vi "TS Manager_wo TS.vi"(11 "notifier":refnum<notifier>) -> ()   [LabVIEW 2025, in "Config Tool.lvlib"]
doc: "This is the main VI for the configuration editor.Copyright 2017 National Instruments Corporation\n\nLicensed under the Apache License, Version 2.0 (the \"License\"); you may not use this file except in compliance with the License. You may obtain a copy of the License at http://www.apache.org/licenses/LICENSE-2.0\nUnless required by applicable law or agreed to in writing, software distributed under the License is distributed on an \"AS IS\" BASIS, WITHOUT WARRANTIES OR CONDITIONS OF ANY KIND, either express or implied. See the License for the specific language governing permissions and limitations under the License."
uses:
  Controls/StateCluster.ctl
  Users/Public/Documents/Sandia National Labs/TSS Plugin/CEF.lvlibp/Repository/CEF_Repository.lvclass
  Users/Public/Documents/Sandia National Labs/TSS Plugin/CEF.lvlibp/Node/NodeRef.ctl
  Users/Public/Documents/Sandia National Labs/TSS Plugin/CEF.lvlibp/Node/CEF_Node.lvclass
  Users/Public/Documents/Sandia National Labs/TSS Plugin/CEF.lvlibp/Node/StandardEvents.ctl
  Controls/FilePaths.ctl
  Users/Public/Documents/Sandia National Labs/TSS Plugin/CEF.lvlibp/glyph manager/glyph manager.ctl
  <vilib>/Utility/config.llb/Config Data RefNum.ctl
  Controls/AddMessage.ctl
  Controls/MoveMessage.ctl
  Users/Public/Documents/Sandia National Labs/TSS Plugin/CEF.lvlibp/hierarchy repo/CEF_HierarchyRepo.lvclass
  Users/Public/Documents/Sandia National Labs/TSS Plugin/System.lvlibp/System/System.lvclass
  Users/Public/Documents/Sandia National Labs/TSS Plugin/CEF.lvlibp/serializable node/CEF_serializable node.lvclass
  ce7dbd15-68e1-444f-b0a0-607e461cde1a.vi
  TestStandUI/Control Globals.vi
  Users/Public/Documents/Sandia National Labs/TSS Plugin/CEF.lvlibp/Node/ReadChildren.vi
  Users/Public/Documents/Sandia National Labs/TSS Plugin/CEF.lvlibp/Node/ReadNodeClass.vi
  Config Tool.lvlib
  C:/Users/Public/Documents/Sandia National Labs/TSS Plugin/CEF.lvlibp/Repository/CEF_Repository.lvclass
  C:/Users/Public/Documents/Sandia National Labs/TSS Plugin/CEF.lvlibp/hierarchy repo/CEF_HierarchyRepo.lvclass
  C:/Users/Public/Documents/Sandia National Labs/TSS Plugin/CEF.lvlibp/Node/CEF_Node.lvclass
  C:/Users/Public/Documents/Sandia National Labs/TSS Plugin/CEF.lvlibp/serializable node/CEF_serializable node.lvclass
  Users/Public/Documents/Sandia National Labs/TSS Plugin/CEF.lvlibp
  <vilib>/Utility/config.llb/NI_LVConfig.lvlib
panel:
  in  "Record":bool
  out "Time":dbl format="%<%H:%M:%S>t"
  in  "Initialize Engines":bool
  in  "File Menu":bool
  in  "TreeView":string(tree)="NID741343233"
  in  "TS Pane":bool
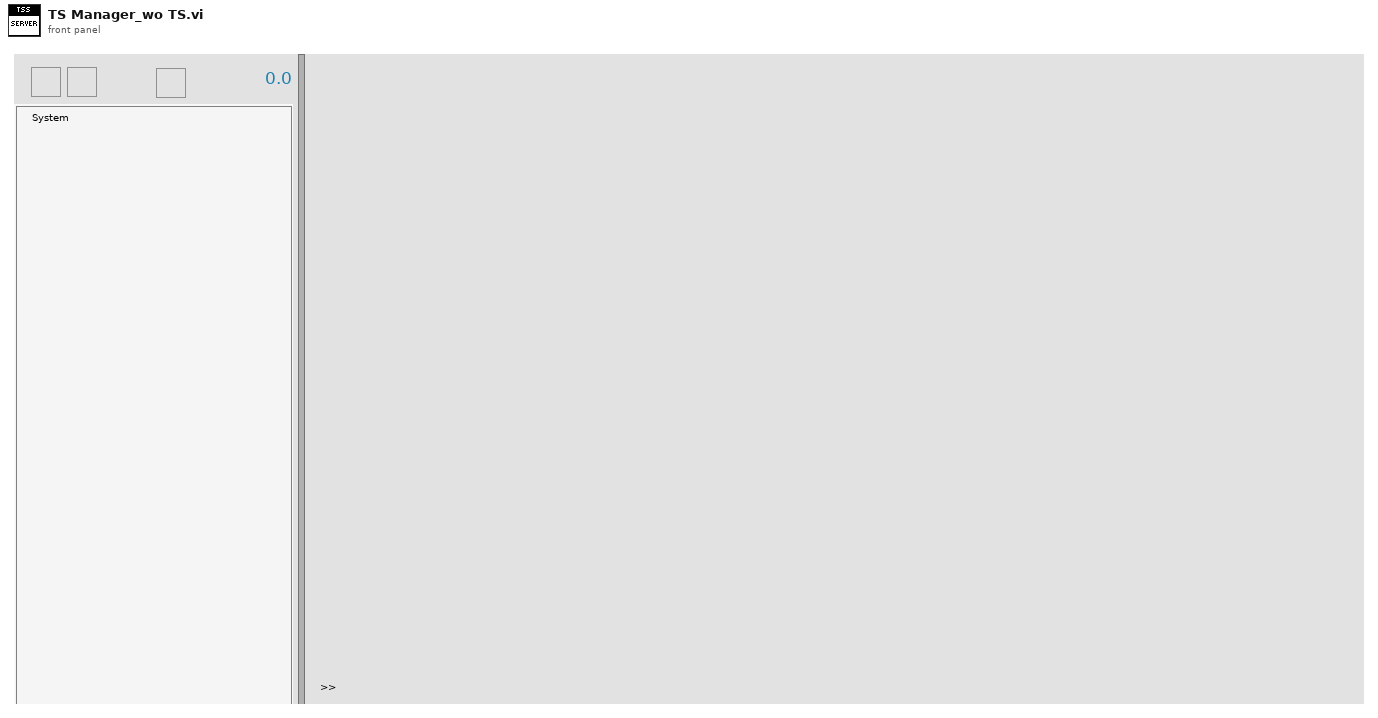
[diagram p1: front panel]
types:
  T1 = typedef "Config Tool.lvlib/StateCluster.ctl" = cluster{"repository":refnum<class "CEF_Repository.lvclass">, "root":T2, "standard events":T3, "paths":T4, "glyph manager":T5, "current path":path, "unsaved changes":bool, "menu":refnum<k9>, "Error Log":refnum<file>, "INI file ref":T6, "Record":bool, "tdms file":refnum<k34>}
  T2 = typedef "CEF.lvlibp/CEF_Node.lvclass/NodeRef.ctl" = refnum<data-value>
  T3 = typedef "CEF.lvlibp/CEF_Node.lvclass/StandardEvents.ctl" = cluster{"user event":refnum<user-event>, "node change":refnum<user-event>, "cache state":refnum<user-event>, "refresh UI":refnum<user-event>, "stop event":refnum<user-event>, "Quit App":refnum<user-event>}
  T4 = typedef "Config Tool.lvlib/FilePaths.ctl" = cluster{"Configuration":path, "Plugin":path, "Glyphs":path, "Data":path, "Error Log":path}
  T5 = typedef "CEF.lvlibp/glyph manager.ctl" = cluster{"search paths":path[], "glyph map":variant, "base glyphs":cluster{"image type":i32, "image depth":i32, "image":u8[], "mask":u8[], "colors":u32[], "Rectangle":cluster{"left":i16, "top":i16, "right":i16, "bottom":i16}}[], "desired overlays":string[]}
  T6 = typedef "NI_LVConfig.lvlib/Config Data RefNum.ctl" = refnum<k1>
  T7 = cluster{"user event":refnum<user-event>, "node change":refnum<user-event>, "cache state":refnum<user-event>, "refresh UI":refnum<user-event>, "stop event":refnum<user-event>, "Quit App":refnum<user-event>}
  T8 = typedef "Config Tool.lvlib/AddMessage.ctl" = cluster{"subNode":string, "Node ID":string}
  T9 = typedef "Config Tool.lvlib/MoveMessage.ctl" = cluster{"node ref":T2, "new parent":T2, "Index":i32}
  T10 = cluster{"Message Name":string, "data string":string}
  T11 = typedef "LVPoint32TypeDef.ctl" = cluster{"Horizontal":i32, "Vertical":i32}
  T12 = cluster{"data name":string, "drag data":variant}[]
  T13 = cluster{"removable":bool, "movable":bool, "duplicate":bool}
  T14 = cluster{"message name":string, "data string":string}
  T15 = enum16{"Start Timer", "Read Time", "Pause", "Resume"}
  T16 = enum16{"open", "open or create", "create or replace", "create", "open (read-only)"}
  T17 = cluster{"search paths":path[], "glyph map":variant, "base glyphs":cluster{"image type":i32, "image depth":i32, "image":u8[], "mask":u8[], "colors":u32[], "Rectangle":cluster{"left":i16, "top":i16, "right":i16, "bottom":i16}}[], "desired overlays":string[]}
  T18 = cluster{"ID":string, "parent ID":string, "node type":string, "text":string, "additional text":string, "glyph":string, "depth":i32, "glyph overlay":string}[]
  T19 = cluster{"ID":string, "parent ID":string, "node type":string, "text":string, "additional text":string, "glyph":string, "depth":i32, "glyph overlay":string}
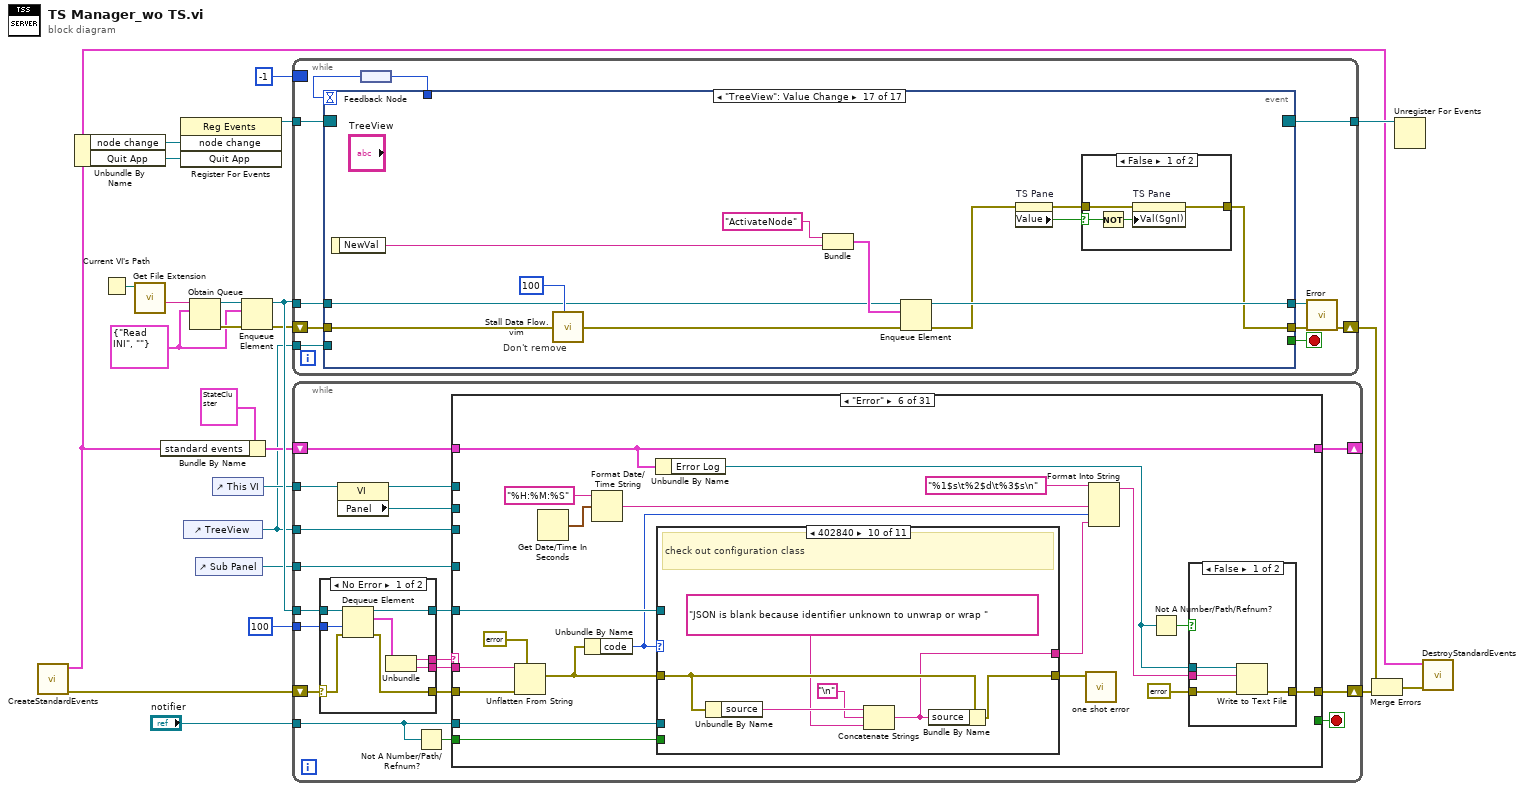
[diagram p0: block diagram]
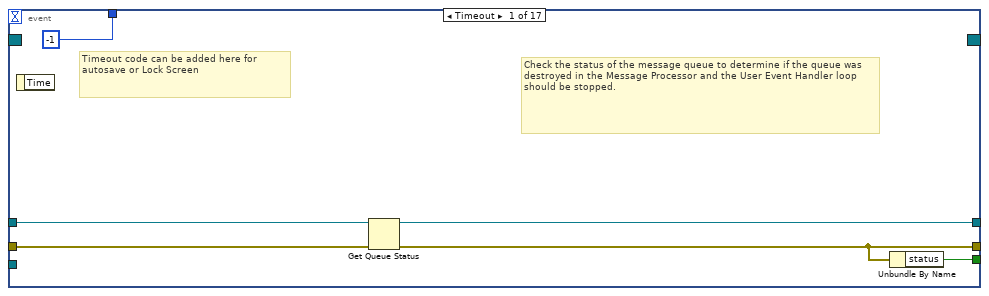
[diagram p2: hidden frame]
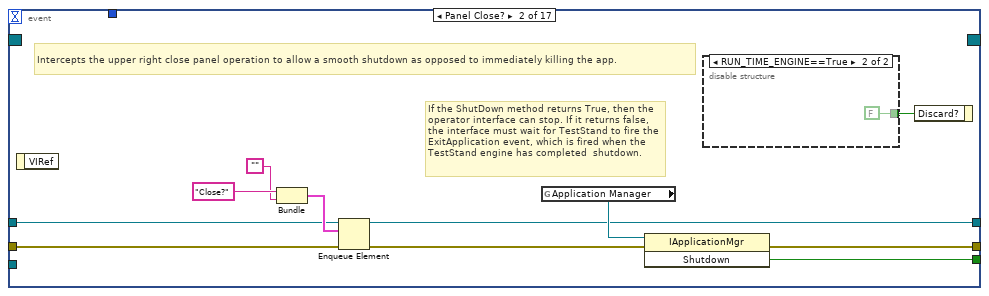
[diagram p3: hidden frame]
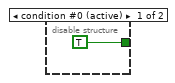
[diagram p4: hidden frame]
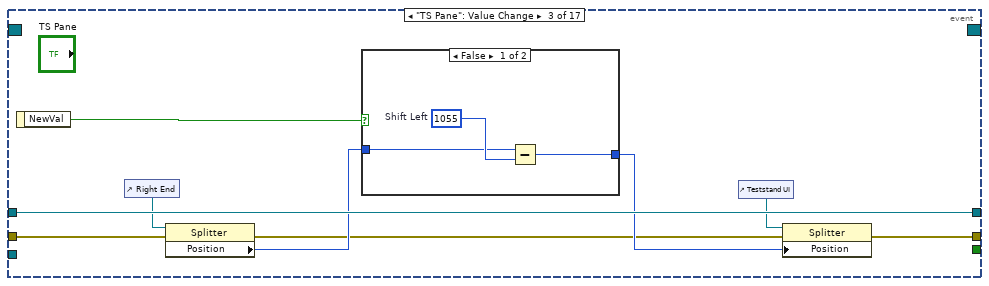
[diagram p5: hidden frame]
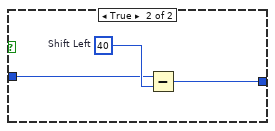
[diagram p6: hidden frame]
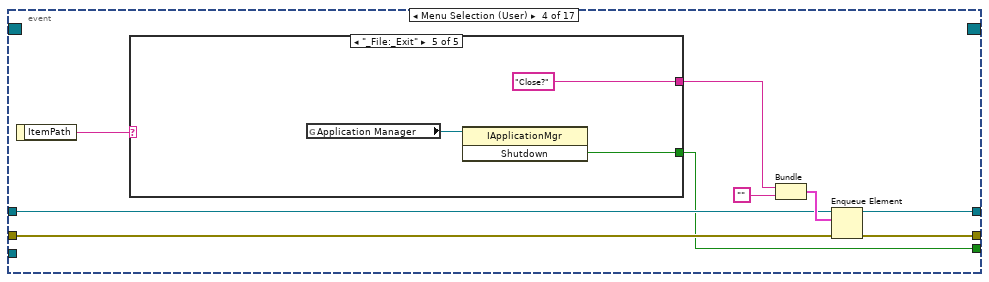
[diagram p7: hidden frame]
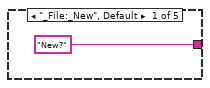
[diagram p8: hidden frame]
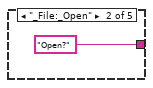
[diagram p9: hidden frame]
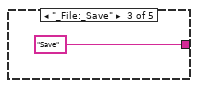
[diagram p10: hidden frame]
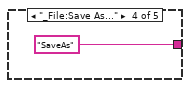
[diagram p11: hidden frame]
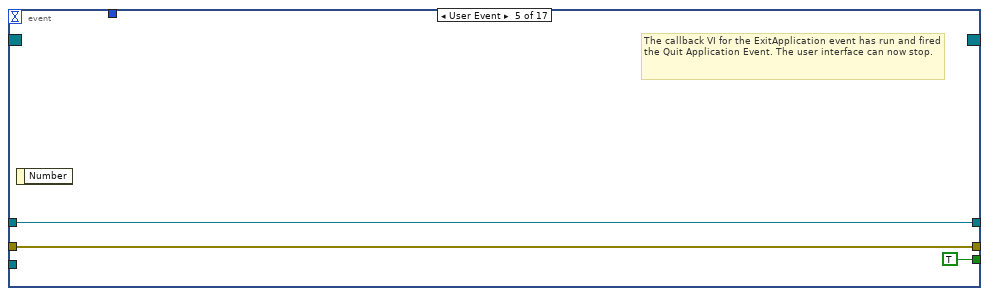
[diagram p12: hidden frame]
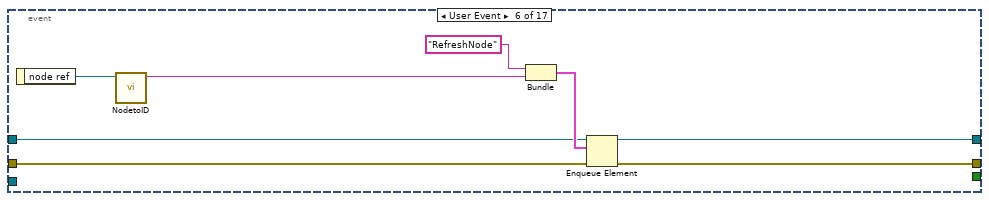
[diagram p13: hidden frame]
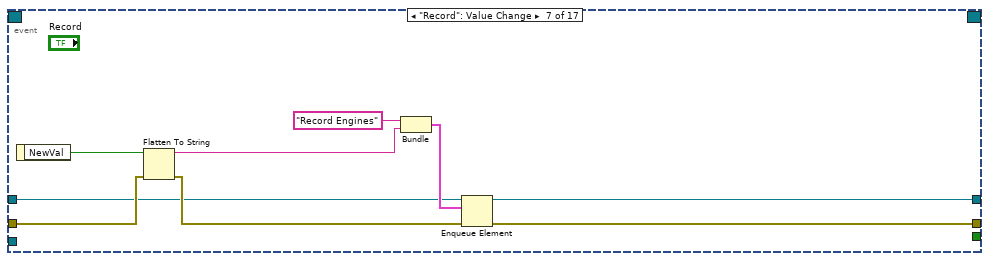
[diagram p14: hidden frame]
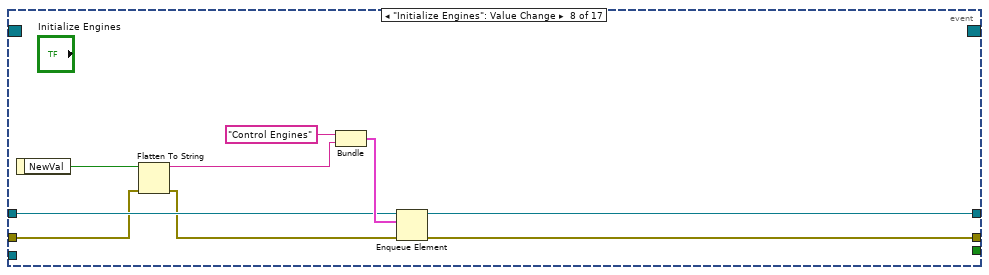
[diagram p15: hidden frame]
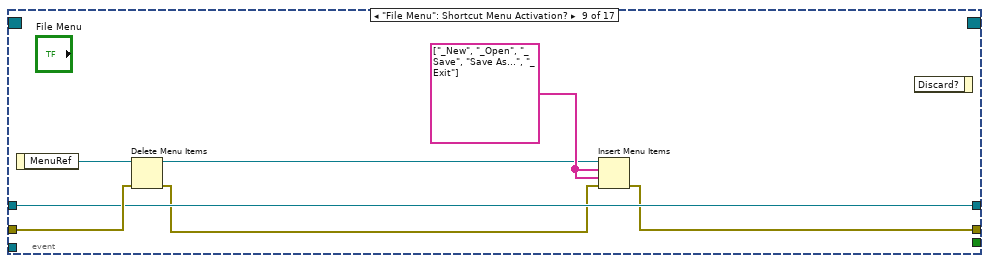
[diagram p16: hidden frame]
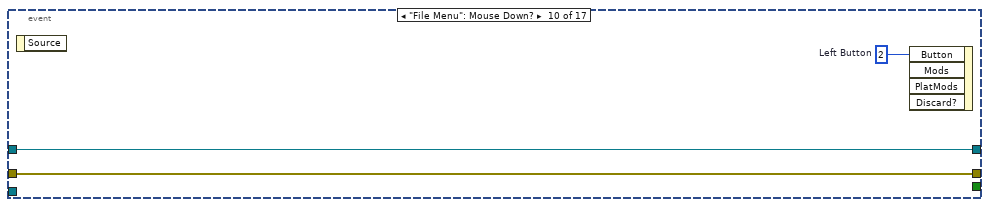
[diagram p17: hidden frame]
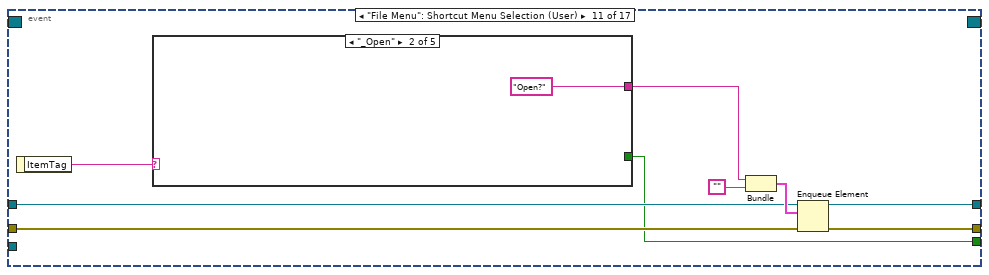
[diagram p18: hidden frame]
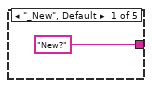
[diagram p19: hidden frame]
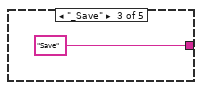
[diagram p20: hidden frame]
diagram:
  w10 = cluster{"message":string, "string":string} {"message"="Read INI", "string"=""}
  n1 = call "CreateStandardEvents.vi"() -> ("error out"=w14:errorcluster, "standard events"=w16:T7)  [unwired: 10 in]
  n2 = Unbundle By Name(w16) -> ("node change"=w15:refnum<user-event>, "Quit App"=w1:refnum<user-event>)
  n3 = Current VI's Path() -> (path=w21:path)
  n4 = call <vilib>:"Get File Extension.vi"("file"=w21) -> ("filename without extension"=w11:string)  [unwired: 6 in, 4 out]
  n5 = Bundle By Name(cluster=T1 {"repository"=refnum, "root"=refnum, "standard events"={"user event"=refnum, "node change"=refnum, "cache state"=refnum, "refresh UI"=refnum, "stop event"=refnum, "Quit App"=refnum}, "paths"={"Configuration"=path "", "Plugin"=path "", "Glyphs"=path "", "Data"=path "", "Error Log"=path ""}, "glyph manager"={"search paths"=[], "glyph map"=variant, "base glyphs"=[], "desired overlays"=[]}, "current path"=path "", "unsaved changes"=FALSE, "menu"=refnum, "Error Log"=refnum, "INI file ref"=refnum, "Record"=FALSE, "tdms file"=refnum} ("state cluster"), "standard events"=w16) -> (w4:T1)
  n6 = register-events(w15, w1) -> (reference out=w2:refnum<event-registration>)  [unwired: 2 in, 1 out]
  n7 = control-ref of="TreeView"() -> (w3:refnum<vi>)
  n8 = Obtain Queue(name (unnamed)=w11, element data type=w10) -> (queue out=w12:refnum<queue>, error out=w13:errorcluster)  [unwired: 3 in, 1 out]
  n9 = control-ref of="Sub Panel"() -> (w5:refnum<vi>)
  n10 = control-ref of="This VI"() -> (w6:refnum<vi>)
  n11 = Enqueue Element(queue=w12, element=w10, error in (no error)=w13) -> (queue out=w9:refnum<queue>, error out=w8:errorcluster)  [unwired: 1 in, 1 out]
  n12 = while "User Interface Event Handler" {
    tunnel: w9 -> [w34]
    tunnel: w3 -> [w29]
    tunnel: w2 -> [w28]
    tunnel: [w27] -> w17
    border: -1 -> [_]
    shift-right: [w31] -> w22
    shift-left: w8 -> [w35]
    stop <- w33 stop-if-true
    n13 = feedback #1() -> (w25:i32)
    n14 = event shown="[16] \"TreeView\": Value Change" {
      selector: w28 -> [_ _ _ _ _ _ _ _ _ _ _ _ _ _ _ _ _]
      dyn-events: [_ _ _ _ _ _ _ _ _ _ _ _ _ _ _ _ _] -> w27
      timeout: w25 -> [_ _ _ _ _ _ _ _ _ _ _ _ _ _ _ _ _]
      tunnel: [w36 w49 _ w71 TRUE ("Shutdown") _ _ _ _ _ w127 _ _ _ _ _ _] -> w33
      tunnel: [w37 w51 w62 w78 w90 w97 w101 w108 w117 w124 w128 w159 w182 w211 w239 w250 w279] -> w32
      tunnel: w35 -> [w38 w45 w57 w72 w90 w91 w103 w110 w123 w124 w129 w150 w181 w210 w237 w251 w290]
      tunnel: w34 -> [w41 w44 w64 w73 w89 w93 w102 w114 w121 w125 w131 w148 w177 w209 w236 w245 w284]
      tunnel: [w40 w43 w64 w77 w89 w92 w100 w113 w121 w125 w130 w148 w176 w209 w236 _ w283] -> w30
      tunnel: w29 -> [_ _ _ _ _ _ _ _ _ _ _ w146 _ _ _ _ _]
      tunnel: [-1 _ _ _ _ _ _ _ _ _ _ _ _ _ _ _ _] -> w26
      event Timeout {
        # "Check the status of the message queue to determine if the queue was destroyed in the Message Processor and the User Event Handler loop should be stopped."
        # "Timeout code can be added here for autosave or Lock Screen"
        n15 = event-data() -> ()  [unwired: 1 in, 1 out]
        n16 = Get Queue Status(queue=w41, error in (no error)=w38) -> (queue out=w40:refnum<queue>, error out=w37:errorcluster)  [unwired: 1 in, 6 out]
        n17 = Unbundle By Name(w37) -> ("status"=w36:bool)
      }
      event Panel Close? {
        # "If the ShutDown method returns True, then the operator interface can stop. If it returns false, the interface must wait for TestStand to fire the ExitApplication event, which is fired when the TestStand engine has completed  shutdown."
        # "Intercepts the upper right close panel operation to allow a smooth shutdown as opposed to immediately killing the app."
        n18 = event-data() -> ()  [unwired: 1 in, 1 out]
        n19 = Bundle("Close?", "") -> (w48:cluster{string, string})  [unwired: 1 in]
        n20 = Enqueue Element(queue=w44, element=w48, error in (no error)=w45) -> (queue out=w43:refnum<queue>, error out=w42:errorcluster)  [unwired: 1 in, 1 out]
        n21 = global read "Control Globals.vi" "Application Manager"() -> (w50:refnum<k7>)
        n22 = global read "Control Globals.vi" "Application Manager"() -> (w52:refnum<k7>)
        n23 = invoke class="IApplicationMgr" method="Shutdown"(reference=w50, error in=w42) -> ()  [unwired: 1 in, 3 out]
        n24 = invoke class="IApplicationMgr" method="Shutdown"(reference=w52) -> (error out=w51:errorcluster, "Shutdown"=w49:bool)  [unwired: 2 in, 1 out]
        n25 = disable-structure shown="RUN_TIME_ENGINE==True" {
          disable-tunnel: [TRUE FALSE] -> w53
          frame condition #0 (active) {
          }
          frame condition #1 {
          }
        }
        n26 = event-data("Discard?"=w53) -> ()  [unwired: 1 in, 1 out]
      }
      event "TS Pane": Value Change {
        n27 = event-data() -> ("NewVal"=w60:bool)  [unwired: 1 in]
        n28 = control-ref of="Right End"() -> (w61:refnum<vi>)
        n29 = property class="Splitter"(reference=w61, error in=w57) -> (error out=w56:errorcluster, "Position"=w59:i32)  [unwired: 1 out]
        n30 = case shown="False" w60 {
          tunnel: w59 -> [w66 w69]
          tunnel: [w65 w68] -> w58
          frame False {
            w67 = 1055  # Shift Left
            n31 = Subtract(x=w66, y=w67) -> (x-y=w65:i32)
          }
          frame True {
            w70 = 40  # Shift Left
            n32 = Subtract(x=w69, y=w70) -> (x-y=w68:i32)
          }
        }
        n33 = control-ref of="Teststand UI"() -> (w63:refnum<vi>)
        n34 = property class="Splitter"(reference=w63, error in=w56, "Position"=w58) -> (error out=w62:errorcluster)  [unwired: 1 out]
      }
      event Menu Selection (User) {
        n35 = event-data() -> ("ItemPath"=w79:string)  [unwired: 1 in]
        n36 = case shown="\"_File:_Exit\"" w79 {
          tunnel: ["New?" ("Message Name") "Open?" ("Message Name") "Save" ("Message Name") "SaveAs" ("Message Name") "Close?" ("Message Name")] -> w75
          tunnel: [_ _ _ _ w84] -> w71
          frame "_File:_New", Default {
          }
          frame "_File:_Open" {
          }
          frame "_File:_Save" {
          }
          frame "_File:Save As..." {
          }
          frame "_File:_Exit" {
            n37 = global read "Control Globals.vi" "Application Manager"() -> (w85:refnum<k7>)
            n38 = global read "Control Globals.vi" "Application Manager"() -> (w86:refnum<k7>)
            n39 = invoke class="IApplicationMgr" method="Shutdown"(reference=w85) -> ("Shutdown"=w84:bool)  [unwired: 2 in, 2 out]
            n40 = invoke class="IApplicationMgr" method="Shutdown"(reference=w86) -> ()  [unwired: 2 in, 3 out]
          }
        }
        n41 = Bundle("Message Name"=w75, "") -> (w74:cluster{"Message Name":string, string})  [unwired: 1 in]
        n42 = Enqueue Element(queue=w73, element=w74, error in (no error)=w72) -> (queue out=w77:refnum<queue>, error out=w78:errorcluster)  [unwired: 1 in, 1 out]
      }
      event User Event {
        # "The callback VI for the ExitApplication event has run and fired the Quit Application Event. The user interface can now stop."
        n43 = event-data() -> ()  [unwired: 1 in, 1 out]
      }
      event User Event {
        n44 = event-data() -> ("node ref"=w98:refnum<data-value>)  [unwired: 1 in]
        n45 = call "NodetoID.vi"("node ref"=w98) -> ("ID"=w94:string)  [unwired: 9 in, 1 out]
        n46 = Bundle("message name"="RefreshNode", "ID"=w94) -> (w95:cluster{"message name":string, "ID":string})  [unwired: 1 in]
        n47 = Enqueue Element(queue=w93, element=w95, error in (no error)=w91) -> (queue out=w92:refnum<queue>, error out=w97:errorcluster)  [unwired: 1 in, 1 out]
      }
      event "Record": Value Change {
        n48 = event-data() -> ("NewVal"=w99:bool)  [unwired: 1 in]
        n49 = Flatten To String(anything=w99, error in (no error)=w103) -> (data string=w105:string, error out=w104:errorcluster)  [unwired: 2 in, 1 out]
        n50 = Bundle("Message Name"="Record Engines", "data string"=w105) -> (w107:T10)  [unwired: 1 in]
        n51 = Enqueue Element(queue=w102, element=w107, error in (no error)=w104) -> (queue out=w100:refnum<queue>, error out=w101:errorcluster)  [unwired: 1 in, 1 out]
      }
      event "Initialize Engines": Value Change {
        n52 = event-data() -> ("NewVal"=w112:bool)  [unwired: 1 in]
        n53 = Flatten To String(anything=w112, error in (no error)=w110) -> (data string=w111:string, error out=w109:errorcluster)  [unwired: 2 in, 1 out]
        n54 = Bundle("Message Name"="Control Engines", "data string"=w111) -> (w116:T10)  [unwired: 1 in]
        n55 = Enqueue Element(queue=w114, element=w116, error in (no error)=w109) -> (queue out=w113:refnum<queue>, error out=w108:errorcluster)  [unwired: 1 in, 1 out]
      }
      event "File Menu": Shortcut Menu Activation? {
        w120 = string[] ["_New", "_Open", "_Save", "Save As...", "_Exit"] ("item names")
        n56 = event-data() -> ("MenuRef"=w122:refnum<k9>)  [unwired: 1 in]
        n57 = Delete Menu Items(6:w123, 9:w122) -> (0:w118:errorcluster, 3:w119:refnum<k9>)  [unwired: 2 in]
        n58 = Insert Menu Items(6:w118, 7:w120, 8:w120, 9:w119) -> (0:w117:errorcluster)  [unwired: 2 in, 2 out]
        n59 = event-data() -> ()  [unwired: 2 in, 1 out]
      }
      event "File Menu": Mouse Down? {
        w126 = u16 2  # Left Button
        n60 = event-data() -> ()  [unwired: 1 in, 1 out]
        n61 = event-data("Button"=w126) -> ()  [unwired: 4 in, 1 out]
      }
      event "File Menu": Shortcut Menu Selection (User) {
        n62 = event-data() -> ("ItemTag"=w135:string)  [unwired: 1 in]
        n63 = case shown="\"_Open\"" w135 {
          tunnel: ["New?" ("Message Name") "Open?" ("Message Name") "Save" ("Message Name") "SaveAs" ("Message Name") "Close?" ("Message Name")] -> w133
          tunnel: [_ _ _ _ w141] -> w127
          frame "_New", Default {
          }
          frame "_Open" {
          }
          frame "_Save" {
          }
          frame "Save As..." {
          }
          frame "_Exit" {
            n64 = global read "Control Globals.vi" "Application Manager"() -> (w142:refnum<k7>)
            n65 = global read "Control Globals.vi" "Application Manager"() -> (w143:refnum<k7>)
            n66 = invoke class="IApplicationMgr" method="Shutdown"(reference=w142) -> ("Shutdown"=w141:bool)  [unwired: 2 in, 2 out]
            n67 = invoke class="IApplicationMgr" method="Shutdown"(reference=w143) -> ()  [unwired: 2 in, 3 out]
          }
        }
        n68 = Bundle("Message Name"=w133, "") -> (w132:cluster{"Message Name":string, string})  [unwired: 1 in]
        n69 = Enqueue Element(queue=w131, element=w132, error in (no error)=w129) -> (queue out=w130:refnum<queue>, error out=w128:errorcluster)  [unwired: 1 in, 1 out]
      }
      event "TreeView": Shortcut Menu Activation? {
        n70 = event-data() -> ("MenuRef"=w149:refnum<k9>, "CtlRef"=w162:refnum<vi>, "Coords"=w161:T11)  [unwired: 1 in]
        n71 = invoke class="Tree (strict)" method="Point To Row Column"(reference=w162, "Point"=w161) -> ("Tag"=w160:string)  [unwired: 6 in, 7 out]
        n72 = property class="Tree (strict)"(reference=w146, error in=w150) -> (error out=w147:errorcluster, "Allow Editing Cells"=w145:bool)  [unwired: 1 out]
        n73 = call "IDtoNode.vi"("error in"=w147, "ID"=w160) -> ("error out"=w155:errorcluster, "invalid Id"=w153:bool, "node ref"=w158:refnum<data-value>)  [unwired: 7 in]
        n74 = Not(x=w153) -> (.not. x?=w144:bool)
        n75 = And(x=w144, y=w145) -> (x .and. y?=w152:bool)
        n76 = case shown="True" w152 {
          tunnel: w158 -> [_ w170]
          tunnel: w149 -> [_ w169]
          tunnel: [_ w168] -> w157
          tunnel: [_ w167] -> w156
          tunnel: w155 -> [w164 w166]
          tunnel: [w164 w166] -> w154
          tunnel: [TRUE ("Discard?") FALSE ("Discard?")] -> w151
          frame False {
          }
          frame True {
            n77 = in-place {
              in-place-border: w169 -> [w173]
              in-place-border: [w171] -> w168
              n78 = in-place-dvr #2(w170) -> (w175:refnum<class "CEF_Node.lvclass">, w172:errorcluster)
              n79 = call-dynamic "ShortcutMenu.vi"("error in"=w172, "menu ref in"=w173, "CEF_Node in"=w175) -> ("error out"=w171:errorcluster, "CEF_Node out"=w174:refnum<class "CEF_Node.lvclass">)  [unwired: 6 in, 1 out]
              n80 = in-place-dvr #2(w174) -> (w167:errorcluster)  [unwired: 1 out]
            }
          }
        }
        n81 = Merge Errors(w156, w157, w154) -> (w159:errorcluster)
        n82 = event-data("Discard?"=w151) -> ()  [unwired: 1 in, 1 out]
      }
      event "TreeView": Shortcut Menu Selection (User) {
        n83 = event-data() -> ("ItemPath"=w184:string, "CtlRef"=w187:refnum<vi>, "Coords"=w188:T11)  [unwired: 1 in]
        n84 = invoke class="Tree (strict)" method="Point To Row Column"(reference=w187, "Point"=w188) -> ("Tag"=w183:string)  [unwired: 6 in, 7 out]
        n85 = Match Pattern(string=w184, regular expression=":") -> (before substring=w186:string, after substring=w185:string)  [unwired: 1 in, 2 out]
        n86 = case shown="\"Export\"" w186 {
          selector: w186 -> [w192 _ _ _ _ _]
          tunnel: w185 -> [_ _ _ w202 _ _]
          tunnel: w183 -> [w193 w195 w197 w203 w205 w208]
          tunnel: ["CustomMenuAction" ("Message Name") "RemoveNode" ("Message Name") "Duplicate" ("Message Name") "AddNode" ("Message Name") "Import Engine" ("Message Name") "Export Engine" ("Message Name")] -> w179
          tunnel: [w190 w195 w197 w199 w205 w208] -> w180
          frame Default {
            # "Right click menu"
            n87 = Concatenate Strings(w192, ":" ("string"), w193) -> (w190:string)
          }
          frame "Remove" {
          }
          frame "Duplicate" {
          }
          frame "Add" {
            n88 = Bundle By Name(cluster=T8 {"subNode"="", "Node ID"=""} ("input cluster"), "subNode"=w202, "Node ID"=w203) -> (w200:T8)
            n89 = Flatten To String(anything=w200) -> (data string=w199:string)  [unwired: 3 in, 2 out]
          }
          frame "Import" {
          }
          frame "Export" {
          }
        }
        n90 = Bundle("Message Name"=w179, "Tag"=w180) -> (w178:cluster{"Message Name":string, "Tag":string})  [unwired: 1 in]
        n91 = Enqueue Element(queue=w177, element=w178, error in (no error)=w181) -> (queue out=w176:refnum<queue>, error out=w182:errorcluster)  [unwired: 1 in, 1 out]
      }
      event "TreeView": Drag Starting? {
        n92 = event-data() -> ("Data"=w218:T12, "CtlRef"=w220:refnum<vi>, "Coords"=w219:T11)  [unwired: 1 in]
        n93 = invoke class="Tree (strict)" method="Point To Row Column"(reference=w220, "Point"=w219) -> ("Tag"=w217:string)  [unwired: 6 in, 7 out]
        n94 = call "IDtoNode.vi"("error in"=w210, "ID"=w217) -> ("error out"=w212:errorcluster, "invalid Id"=w216:bool, "node ref"=w215:refnum<data-value>)  [unwired: 7 in]
        n95 = case shown="False" w216 {
          tunnel: w215 -> [w228 _]
          tunnel: [w225 TRUE ("Removable")] -> w213
          tunnel: w212 -> [w224 w234]
          tunnel: [w221 w234] -> w211
          frame False {
            n96 = in-place {
              in-place-border: [w231] -> w227
              in-place-border: w224 -> [w230]
              in-place-border: [w229] -> w223
              n97 = in-place-dvr #3(w228) -> (w233:refnum<class "CEF_Node.lvclass">)  [unwired: 1 out]
              n98 = call-dynamic "EditOptions.vi"("error in"=w230, "CEF_Node in"=w233) -> ("error out"=w229:errorcluster, "edit options"=w231:T13, "CEF_Node out"=w232:refnum<class "CEF_Node.lvclass">)  [unwired: 6 in, 1 out]
              n99 = in-place-dvr #3(w232) -> (w222:errorcluster)  [unwired: 1 out]
            }
            n100 = Unbundle By Name(w227) -> ("movable"=w226:bool)
            n101 = Merge Errors(w222, w223) -> (w221:errorcluster)
            n102 = Not(x=w226) -> (.not. x?=w225:bool)
          }
          frame True {
          }
        }
        n103 = event-data("Data"=w218, "Drag Mode"=enum32{"copy or move", "copy only", "move only"}."move only", "Discard?"=w213) -> ()  [unwired: 1 in, 1 out]
      }
      event "TreeView": event type 3.0.xa000003a {
        n104 = event-data() -> ("CtlRef"=w244:refnum<vi>, "Coords"=w241:T11)  [unwired: 1 in]
        n105 = invoke class="Tree (strict)" method="Point To Row Column"(reference=w244, "Point"=w241) -> (reference out=w243:refnum<vi>, "Tag"=w242:string)  [unwired: 6 in, 6 out]
        n106 = call "ValidDragDrop.vi"("error in"=w237, "Reorder"=TRUE, "drag over"=w242, "Tree Ref in"=w243) -> ("Error Out"=w239:errorcluster, "Accepted"=w240:bool)  [unwired: 6 out]
        n107 = event-data("Accepted?"=w240) -> ()  [unwired: 1 in, 1 out]
      }
      event "TreeView": Drop {
        n108 = event-data() -> ("CtlRef"=w262:refnum<vi>, "Coords"=w261:T11)  [unwired: 1 in]
        n109 = invoke class="Tree (strict)" method="Point To Row Column"(reference=w262, "Point"=w261) -> (reference out=w260:refnum<vi>, "Tag"=w257:string)  [unwired: 6 in, 6 out]
        n110 = call "ValidDragDrop.vi"("error in"=w251, "Reorder"=TRUE, "drag over"=w257, "Tree Ref in"=w260) -> ("Error Out"=w249:errorcluster, "Accepted"=w255:bool, "Drag"=w259:string, "Tree Ref out"=w264:refnum<vi>, "Moved Node"=w253:refnum<data-value>, "Position"=w252:i32, "Parent Node"=w254:refnum<data-value>, "Parent"=w256:string)
        n111 = case shown="True" w255 {
          tunnel: w259 -> [_ w276]
          tunnel: w264 -> [_ w278]
          tunnel: [_ TRUE] -> w263
          tunnel: w256 -> [_ w275]
          tunnel: w253 -> [_ w274]
          tunnel: w254 -> [_ w273]
          tunnel: w252 -> [_ w272]
          tunnel: ["Idle" ("message name") "Move" ("message name")] -> w248
          tunnel: [_ w267] -> w247
          frame False {
          }
          frame True {
            n112 = invoke class="Tree (strict)" method="Edit Tree Items.Move Item"(reference=w278, "tag"=w276, "New Parent"=w275, "New Position"=0, "Carry Children"=FALSE ("Carry Children?")) -> ()  [unwired: 2 in, 7 out]
            n113 = Bundle By Name(cluster=T9 {"node ref"=refnum, "new parent"=refnum, "Index"=0}, "Index"=w272, "node ref"=w274, "new parent"=w273) -> (w269:T9)
            n114 = Flatten To String(anything=w269) -> (data string=w267:string)  [unwired: 3 in, 2 out]
          }
        }
        n115 = Bundle("message name"=w248, "data string"=w247) -> (w246:T14)  [unwired: 1 in]
        n116 = Enqueue Element(queue=w245, element=w246, error in (no error)=w249) -> (error out=w250:errorcluster)  [unwired: 1 in, 2 out]
        n117 = event-data("Accepted?"=w263) -> ()  [unwired: 1 in, 1 out]
      }
      event "TreeView": Value Change {
        # "Don't remove"
        n118 = event-data() -> ("NewVal"=w286:string)  [unwired: 1 in]
        n119 = call "Stall Data Flow.vim"("value in"=w290, "milliseconds to wait"=u32 100) -> ("value out"=w289:errorcluster)  [unwired: 1 out]
        n120 = Bundle("Message Name"="ActivateNode", "NewVal"=w286) -> (w285:cluster{"Message Name":string, "NewVal":string})  [unwired: 1 in]
        n121 = Enqueue Element(queue=w284, element=w285, error in (no error)=w289) -> (queue out=w283:refnum<queue>, error out=w282:errorcluster)  [unwired: 1 in, 1 out]
        n122 = property on="TS Pane" class="Bool (strict)"(error in=w282) -> (error out=w280:errorcluster, "Value"=w281:bool)  [unwired: 1 in, 1 out]
        n123 = case shown="False" w281 {
          selector: w281 -> [w292 _]
          tunnel: w280 -> [w294 w295]
          tunnel: [w293 w295] -> w279
          frame False {
            n124 = Not(x=w292) -> (.not. x?=w291:bool)
            n125 = property on="TS Pane" class="Bool (strict)"(error in=w294, "Val(Sgnl)"=w291) -> (error out=w293:errorcluster)  [unwired: 1 in, 1 out]
          }
          frame True {
          }
        }
      }
    }
    n126 = feedback-in #1(w26) -> ()
    n127 = call "Error.vi"("error in (no error)"=w32, "main queue"=w30) -> ("error out"=w31:errorcluster)  [unwired: 9 in]
  }
  n128 = while "Message Processor" {
    shift-right: [w312] -> _
    shift-left: w4 -> [w313]
    tunnel: w9 -> [w308]
    shift-right: [w299] -> w24
    shift-left: w14 -> [w304]
    tunnel: "notifier" -> [w310]
    tunnel: 100 ("timeout (1 ms)") -> [w306]
    tunnel: w6 -> [w298]
    tunnel: w3 -> [w301]
    tunnel: w5 -> [w300]
    stop <- w305 stop-if-true
    n129 = case shown="No Error" w304 {
      selector: w304 -> [w317 w324]
      tunnel: [w321 _] -> w309
      tunnel: w308 -> [w320 w325]
      tunnel: [w319 w325] -> w307
      tunnel: w306 -> [w318 _]
      tunnel: [w315 "Error" ("message")] -> w303
      tunnel: [w314 w323] -> w302
      frame No Error {
        n130 = Dequeue Element(queue=w320, timeout in ms (-1)=w318, error in (no error)=w317) -> (queue out=w319:refnum<queue>, element=w316:cluster{"message":string, "string":string}, error out=w321:errorcluster)  [unwired: 1 out]
        n131 = Unbundle(w316) -> ("message"=w315:string, "string"=w314:string)
      }
      frame Error {
        n132 = Flatten To String(anything=w324) -> (data string=w323:string)  [unwired: 3 in, 2 out]
      }
    }
    n133 = property class="VI"(reference=w298) -> (reference out=w297:refnum<vi>, "Panel"=w296:refnum<vi>)  [unwired: 1 in, 1 out]
    n134 = Not A Number/Path/Refnum?(number/path/refnum=w310) -> (NaN/Path/Refnum?=w311:bool)
    n135 = case shown="\"Error\"" w303 {
      selector: w303 -> [_ _ _ _ _ _ w549 _ _ _ _ w610 _ _ _ _ _ _ _ _ _ _ _ _ _ _ _ _ _ _ _]
      tunnel: w302 -> [_ _ _ _ _ w481 _ _ _ _ _ _ w634 _ _ _ _ w816 w828 w863 w925 w941 w975 w994 w1039 w1055 _ w1079 w1110 w1179 w1217]
      tunnel: w309 -> [w327 w334 w368 w395 w419 w482 w553 w560 w574 w587 w600 w612 w642 w670 w738 w776 w795 w817 w827 w857 w934 w945 w972 w992 w1036 w1054 w1069 w1080 w1115 w1180 w1218]
      tunnel: [w327 w338 w366 w386 w412 w484 w546 w554 w575 w582 w600 w614 w632 w675 w741 w778 w795 w802 w837 w864 w920 w938 w959 w997 w1031 w1057 w1069 w1074 w1118 w1168 w1214] -> w299
      tunnel: [w326 w349 w365 w404 w415 w483 w547 w570 w580 w596 w599 w603 w648 w690 w745 w777 w794 w825 w832 w862 w935 w939 w977 w1001 w1034 w1059 w1068 w1072 w1119 w1186 w1212] -> w312
      tunnel: w313 -> [w326 w347 w365 w391 w416 w483 w547 w570 w580 w596 w599 w603 w647 w691 w746 w780 w794 w824 w833 w862 w932 w937 w978 w1001 w1033 w1056 w1068 w1073 w1120 w1186 w1213]
      tunnel: w307 -> [_ w337 w371 w400 w414 w474 _ w563 w572 w586 _ w607 w643 w673 _ _ _ w798 _ w861 _ _ _ w998 w1023 w1049 _ _ w1122 w1171 w1211]
      tunnel: w310 -> [_ w344 w369 w393 w421 w472 _ _ _ _ _ _ w644 _ _ _ _ _ _ w855 _ _ w963 _ _ w1041 _ _ _ w1181 _]
      tunnel: w311 -> [_ w342 w370 w392 w420 w471 _ _ _ _ _ _ w635 w671 _ _ _ _ _ _ _ _ w964 _ _ _ _ _ _ w1169 _]
      tunnel: [_ _ _ _ _ _ _ _ _ TRUE ("Exit") _ _ _ _ _ _ _ _ _ _ _ _ _ _ _ _ _ _ _ _ _] -> w305
      tunnel: w297 -> [_ _ _ w397 w417 _ w544 _ _ w581 _ _ _ _ _ _ _ _ _ _ _ _ w965 _ _ _ _ _ _ _ _]
      tunnel: w301 -> [_ w331 _ w387 w418 _ _ _ _ _ _ _ _ _ _ _ _ w796 w826 w858 w918 w936 w968 _ _ w1045 _ _ _ w1182 w1210]
      tunnel: w300 -> [_ _ _ _ _ _ _ _ _ w592 _ _ _ _ _ _ _ _ _ _ _ _ w967 w991 _ _ _ _ _ _ _]
      tunnel: w296 -> [_ _ _ _ _ _ _ w568 _ w591 _ _ _ _ _ _ _ _ _ _ _ _ _ w990 _ _ _ _ _ _ _]
      frame "------------Generic Operations------------" {
        # "Dummy case to add a seperation in the Case Structure menu"
      }
      frame "Read INI" {
        w335 = "Test Config.ini"
        n136 = Bundle("Initialize", "") -> (w340:cluster{string, string})  [unwired: 1 in]
        n137 = Enqueue Element(queue=w337, element=w340, error in (no error)=w334) -> (error out=w333:errorcluster)  [unwired: 1 in, 2 out]
        n138 = case shown="False" w342 {
          tunnel: w344 -> [w356 _]
          tunnel: w333 -> [w353 w357]
          tunnel: [w352 w357] -> w330
          tunnel: w335 -> [w351 _]
          frame False {
            n139 = Bundle("notification"="Read INI", w351) -> (w354:cluster{"notification":string, string})  [unwired: 1 in]
            n140 = Send Notification(notification=w354, notifier=w356, error in (no error)=w353) -> (error out=w352:errorcluster)  [unwired: 1 out]
          }
          frame True {
          }
        }
        n141 = invoke class="Tree (strict)" method="Edit Tree Items.Delete"(reference=w331, "Delete Children"=TRUE ("Delete Children?")) -> (reference out=w329:refnum<vi>)  [unwired: 3 in, 4 out]
        n142 = call <vilib>:"Application Directory.vi"() -> ("Application Directory"=w346:path)
        n143 = Build Path(base path=w346, name or relative path=w335) -> (appended path=w350:path)
        n144 = invoke class="Tree (strict)" method="Custom Item Symbols.Revert Symbols"(reference=w329, error in=w330) -> (error out=w328:errorcluster)  [unwired: 1 in, 2 out]
        n145 = call "Read INI File.vi"("INI File"=w350) -> ("File paths"=w345:T4, "INI refnum"=w348:T6)  [unwired: 8 in, 1 out]
        n146 = Unbundle By Name(w345) -> ("Error Log"=w343:path)
        n147 = call "Log Error.vi"("Error In"=w328, "Log Path"=w343) -> ("Error Out"=w338:errorcluster, "Log refnum out"=w336:refnum<file>)  [unwired: 8 in]
        n148 = Bundle By Name(cluster=w347, "INI file ref"=w348, "paths"=w345, "Error Log"=w336) -> (w349:T1)
      }
      frame "Initialize" {
        n149 = case shown="False" w370 {
          tunnel: w369 -> [w377 _]
          tunnel: w368 -> [w374 w378]
          tunnel: [w373 w378] -> w367
          frame False {
            n150 = Bundle("notification"="Initialize", "") -> (w375:cluster{"notification":string, string})  [unwired: 1 in]
            n151 = Send Notification(notification=w375, notifier=w377, error in (no error)=w374) -> (error out=w373:errorcluster)  [unwired: 1 out]
          }
          frame True {
          }
        }
        n152 = Bundle("Start Application", "") -> (w364:cluster{string, string})  [unwired: 1 in]
        n153 = Enqueue Element(queue=w371, element=w364, error in (no error)=w367) -> (error out=w361:errorcluster)  [unwired: 1 in, 2 out]
        n154 = property on="TS Pane" class="Bool (strict)"(error in=w361, "Val(Sgnl)"=FALSE ("Value (Signaling)")) -> (error out=w359:errorcluster)  [unwired: 1 in, 1 out]
        n155 = property on="Record" class="Bool (strict)"(error in=w359, "Value"=FALSE ("Record")) -> (error out=w366:errorcluster)  [unwired: 1 in, 1 out]
      }
      frame "Start Application" {
        w396 = TRUE ("Front Panel Window:Is Frontmost")
        n156 = Unbundle By Name(w391) -> ("paths.Glyphs"=w390:path)
        n157 = Bundle("New", "") -> (w403:cluster{string, string})  [unwired: 1 in]
        n158 = Enqueue Element(queue=w400, element=w403, error in (no error)=w395) -> (error out=w394:errorcluster)  [unwired: 1 in, 2 out]
        n159 = case shown="False" w392 {
          tunnel: w393 -> [w410 _]
          tunnel: w394 -> [w407 w411]
          tunnel: [w406 w411] -> w388
          frame False {
            n160 = Bundle("notification"="Start", "") -> (w408:cluster{"notification":string, string})  [unwired: 1 in]
            n161 = Send Notification(notification=w408, notifier=w410, error in (no error)=w407) -> (error out=w406:errorcluster)  [unwired: 1 out]
          }
          frame True {
          }
        }
        n162 = property class="VI"(reference=w397, "Front Panel.TitleBarVis"=w396, "Front Panel.IsFrontmost"=w396) -> (reference out=w399:refnum<vi>, error out=w398:errorcluster)  [unwired: 1 in]
        n163 = invoke class="VI" method="Default Vals.Reinit All"(reference=w399, error in=w398) -> (reference out=w383:refnum<vi>)  [unwired: 1 in, 2 out]
        n164 = call "create glyph manager.vi"("error in"=w388, "tree ref (for default symbols)"=w387) -> ("error out"=w382:errorcluster, "glyph manager"=w381:T17)  [unwired: 8 in]
        n165 = call "update tree control.vi"("error in"=w382, "tree reference"=w387, "glyph manager in"=w381) -> ("error out"=w379:errorcluster, "glyph manager out"=w380:T17)  [unwired: 7 in]
        n166 = call "add search path.vi"("error in"=w379, "search path"=w390, "glyph manager in"=w380) -> ("error out"=w386:errorcluster, "glyph manager out"=w389:T17)  [unwired: 7 in]
        n167 = Current VI's Menubar() -> (w385:refnum<k9>)
        n168 = call "MenuOptions.vi"("VI ref"=w383, "menu ref in"=w385) -> ("menu ref out"=w384:refnum<k9>)  [unwired: 8 in, 1 out]
        n169 = Bundle By Name(cluster=w391, "glyph manager"=w389, "menu"=w384) -> (w404:T1)
      }
      frame "", "Idle" {
        n170 = case shown="True" w420 {
          tunnel: w421 -> [_ _]
          tunnel: w419 -> [w423 w436]
          tunnel: [w423 w432] -> w413
          tunnel: w418 -> [_ w425]
          tunnel: w417 -> [_ w434]
          tunnel: w416 -> [w422 w437]
          tunnel: [w422 w437] -> w415
          tunnel: w414 -> [_ w431]
          frame False {
          }
          frame True {
            n171 = Unbundle By Name(w437) -> ("current path"=w438:path, "root"=w428:T2, "Record"=w427:bool, "tdms file"=w424:refnum<k34>)
            n172 = property class="Tree (strict)"(reference=w425, error in=w436) -> (reference out=w443:refnum<vi>, error out=w435:errorcluster, "All Tags"=w445:string[], "NumRows"=w442:u32)
            n173 = property class="NISE_CEF_Node"(reference=w428) -> ("DataAccess:Children"=w430:refnum<data-value>[])  [unwired: 1 in, 2 out]
            n174 = Array Size(array=w445) -> (size(s)=w441:i32)
            n175 = To Unsigned Long Integer(number=w441) -> (unsigned 32bit integer=w444:u32)
            n176 = Path To String(path=w438) -> (string=w439:string)
            n177 = Greater Or Equal?(x=w444, y=w442) -> (x >= y?=w440:bool)
            n178 = property class="VI"(reference=w434, "Front Panel.Title"=w439) -> ()  [unwired: 1 in, 2 out]
            n179 = Index Array(array=w430) -> (element=w429:refnum<data-value>)  [unwired: 1 in]
            n180 = property class="Tree (strict)"(reference=w443, error in=w435, "VScrollVis"=w440) -> (error out=w433:errorcluster)  [unwired: 1 out]
            n181 = property class="NISE_CEF_Node"(reference=w429) -> ("DataAccess:Children"=w426:refnum<data-value>[])  [unwired: 1 in, 2 out]
            n182 = case shown="True" w427 {
              tunnel: w433 -> [w446 w454]
              tunnel: [w446 w453] -> w432
              tunnel: w431 -> [_ w452]
              tunnel: w426 -> [_ w451]
              tunnel: w425 -> [_ w450]
              tunnel: w424 -> [_ w449]
              frame False {
              }
              frame True {
                n183 = for {
                  tunnel: w451 -> [w460] mode=indexing
                  shift-right: [w458] -> w453
                  shift-left: w454 -> [w459]
                  tunnel: w450 -> [w457]
                  tunnel: w452 -> [w456]
                  tunnel: w449 -> [w455]
                  n184 = in-place {
                    in-place-border: w459 -> [w464]
                    in-place-border: [w465] -> w458
                    in-place-border: w457 -> [w467]
                    in-place-border: w456 -> [w462]
                    in-place-border: w455 -> [w461]
                    n185 = in-place-dvr #4(w460) -> (w468:refnum<class "CEF_Node.lvclass">)  [unwired: 1 out]
                    n186 = call-dynamic "MenuHandler.vi"("tree control"=w467, "main queue"=w462, "error in"=w464, "parameters"=w461, "menu string"="Record", "CEF_Node in"=w468) -> ("error out"=w465:errorcluster, "CEF_Node out"=w466:refnum<class "CEF_Node.lvclass">)  [unwired: 2 in, 2 out]
                    n187 = in-place-dvr #4(w466) -> ()  [unwired: 2 out]
                  }
                }
                n188 = call "Timing FGV.vi"("Timer Mode"=T15."Read Time") -> ("Elapsed Time (s.ms)"=→"Time":dbl)  [unwired: 8 in, 2 out]
              }
            }
          }
        }
        n189 = call <vilib>:"Unset Busy.vi"("error in (no error)"=w413) -> ("error out"=w412:errorcluster)  [unwired: 10 in]
      }
      frame "Error" {
        n190 = Unflatten From String(type=errorcluster {"status"=FALSE, "code"=0, "source"=""} ("error out"), binary string=w481, error in (no error)=w482) -> (value=w479:errorcluster)  [unwired: 2 in, 2 out]
        n191 = Get Date/Time In Seconds() -> (seconds since 1Jan1904=w487:timestamp)
        n192 = Unbundle By Name(w479) -> ("code"=w470:i32)
        n193 = Format Date/Time String(time format string (%c)="%H:%M:%S", seconds (now)=w487) -> (date/time string=w478:string)  [unwired: 1 in]
        n194 = Unbundle By Name(w483) -> ("Error Log"=w477:refnum<file>)
        n195 = case shown="402840" w470 {
          tunnel: w479 -> [w494 w496 w499 w506 w509 w511 w516 w524 w525 w530 w535]
          tunnel: [w495 w497 w501 w505 w508 w512 w514 w521 w526 w528 w533] -> w469
          tunnel: w474 -> [_ _ _ _ _ _ _ _ _ _ w543]
          tunnel: [w494 _ w498 w504 w507 w510 w513 _ w525 w527 w534] -> w473
          tunnel: w472 -> [_ _ _ _ _ _ _ _ _ _ w536]
          tunnel: w471 -> [_ _ _ _ _ _ _ _ _ _ _]
          frame 538504, 538505 {
            n196 = Unbundle By Name(w494) -> ("source"=w495:string)
          }
          frame Default {
            n197 = call <vilib>:"Simple Error Handler.vi"("error in (no error)"=w496) -> ()  [unwired: 4 in, 5 out]
            n198 = Unbundle By Name(w496) -> ("source"=w497:string)
          }
          frame -2147220623, -2147220621, -2147220364, 56, 63, 537053 {
            n199 = Unbundle By Name(w499) -> ("source"=w503:string)
            n200 = Concatenate Strings(w503, "\n", "*Note : Problem communicating with remote device.  Make sure a valid device is selected and that the IP address is correct.\n" ("message")) -> (w501:string)
            n201 = Bundle By Name(cluster=w499, "source"=w501) -> (w498:errorcluster)
          }
          frame 1000 {
            w505 = "Invoke error : Abort VI at Subpanel." ("message")
            n202 = Bundle By Name(cluster=w506, "source"=w505) -> (w504:errorcluster)
          }
          frame 1003 {
            w508 = "Dev Error: The Ui.vi for the selected class is broken." ("message")
            n203 = Bundle By Name(cluster=w509, "source"=w508) -> (w507:errorcluster)
          }
          frame 1, 91, 1556, 5001 {
            w512 = "Make sure Variant to data." ("message")
            n204 = Bundle By Name(cluster=w511, "source"=w512) -> (w510:errorcluster)
          }
          frame 15550 {
            n205 = Unbundle By Name(w516) -> ("source"=w518:string)
            n206 = Concatenate Strings(w518, "\n", "*Note : The System does not yet have a configuration to download. Create or open a configuration and download it to the System" ("message")) -> (w514:string)
            n207 = Bundle By Name(cluster=w516, "source"=w514) -> (w513:errorcluster)
          }
          frame -375006, 537549, 538500 {
            n208 = Unbundle By Name(w524) -> ("source"=w520:string)
            n209 = Concatenate Strings(w520, "\n", "*Note : Invalid configuration when opening config file. Check out if it existed or both tags and class names are correct." ("message")) -> (w521:string)
            n210 = Bundle By Name(cluster=w524, "source"=w521) -> (w523:errorcluster)
            n211 = call <vilib>:"Simple Error Handler.vi"("error in (no error)"=w523) -> ()  [unwired: 4 in, 5 out]
          }
          frame 42..44 {
            # "42 : Node Invalid\n43 : Engine unInitialized\n44 : JSON to LVobject"
            n212 = Unbundle By Name(w525) -> ("source"=w526:string)
          }
          frame 402840 {
            # "check out configuration class"
            n213 = Unbundle By Name(w530) -> ("source"=w532:string)
            n214 = Concatenate Strings(w532, "\n", "JSON is blank because identifier unknown to unwrap or wrap " ("message")) -> (w528:string)
            n215 = Bundle By Name(cluster=w530, "source"=w528) -> (w527:errorcluster)
          }
          frame -17006 {
            w533 = "starting application.\nPlease restart LabVIEW program" ("format string")
            # "Teststand UI starting Error"
            n216 = Bundle("Message Name"="Close?", "") -> (w540:cluster{"Message Name":string, string})  [unwired: 1 in]
            n217 = Bundle("notification"="Done", variant) -> (w539:cluster{"notification":string, variant})  [unwired: 1 in]
            n218 = Enqueue Element(queue=w543, element=w540) -> ()  [unwired: 2 in, 3 out]
            n219 = Send Notification(notification=w539, notifier=w536) -> ()  [unwired: 1 in, 2 out]
            n220 = Bundle By Name(cluster=w535, "source"=w533) -> (w534:errorcluster)
          }
        }
        n221 = call "one shot error.vi"("error in"=w473) -> ()  [unwired: 11 in]
        n222 = Format Into String(format string="%1$s\t%2$d\t%3$s\n", w478, w470, w469) -> (resulting string=w485:string)  [unwired: 2 in, 1 out]
        n223 = Not A Number/Path/Refnum?(number/path/refnum=w477) -> (NaN/Path/Refnum?=w476:bool)
        n224 = case shown="False" w476 {
          tunnel: w485 -> [w492 _]
          tunnel: [w491 w493] -> w484
          tunnel: w477 -> [w490 _]
          tunnel: errorcluster {"status"=FALSE, "code"=0, "source"=""} ("error in") -> [w489 w493]
          frame False {
            n225 = Write to Text File(file (use dialog)=w490, text=w492, error in=w489) -> (error out=w491:errorcluster)  [unwired: 1 in, 2 out]
          }
          frame True {
          }
        }
      }
      frame "Missing Message Handler", Default {
        # "Call this case if a message is received that is not handled by any other case. Typically this is a programming error as a result of a typo or unhandled message/missing message handler."
        n226 = property class="VI"(reference=w544) -> (reference out=w545:refnum<vi>, "Name"=w551:string)  [unwired: 1 in, 1 out]
        n227 = Format Into String(format string="DevError: Missing message handler for '%s\" message." ("message"), w549) -> (resulting string=w548:string)  [unwired: 2 in, 1 out]
        n228 = call <vilib>:"Unset Busy.vi"("VI reference (current VI)"=w545) -> ()  [unwired: 10 in, 1 out]
        n229 = call "CEF_error generator.vi"("error in"=w553, "source"=w551, "append error message"=w548, "error code (0)"=538505) -> ("error out"=w546:errorcluster)  [unwired: 5 in]
      }
      frame "Close" {
        w558 = FALSE  # Reset
        n230 = Flatten To String(anything=w558, error in (no error)=w560) -> (data string=w557:string, error out=w559:errorcluster)  [unwired: 2 in, 1 out]
        n231 = Bundle("Control Engines", "data string"=w557) -> (w561:cluster{string, "data string":string})  [unwired: 1 in]
        n232 = Enqueue Element(queue=w563, element=w561, error in (no error)=w559) -> (queue out=w556:refnum<queue>, error out=w564:errorcluster)  [unwired: 1 in, 1 out]
        n233 = Bundle("Write INI File", "") -> (w567:cluster{string, string})  [unwired: 1 in]
        n234 = Enqueue Element(queue=w556, element=w567, error in (no error)=w564) -> (error out=w555:errorcluster)  [unwired: 1 in, 2 out]
        n235 = property class="Pnl"(reference=w568, error in=w555, "DeferPanUpdts"=TRUE ("Defer Panel Updates")) -> (error out=w554:errorcluster)  [unwired: 1 out]
      }
      frame "Write INI File" {
        n236 = Unbundle By Name(w580) -> ("INI file ref"=w571:T6, "paths"=w579:T4)
        n237 = Bundle("Shutdown", "") -> (w578:cluster{string, string})  [unwired: 1 in]
        n238 = Enqueue Element(queue=w572, element=w578, error in (no error)=w574) -> (error out=w573:errorcluster)  [unwired: 1 in, 2 out]
        n239 = call "Write INI File.vi"("error in"=w573, "File path"=w579, "INI refnum"=w571) -> ("error out"=w575:errorcluster)  [unwired: 8 in]
      }
      frame "Shutdown" {
        # "close root DVR"
        n240 = Release Queue(queue=w586, error in (no error)=w587) -> (error out=w585:errorcluster)  [unwired: 1 in, 2 out]
        n241 = property class="Pnl"(reference=w591, "DeferPanUpdts"=FALSE ("Defer Panel Updates")) -> ()  [unwired: 1 in, 2 out]
        n242 = Unbundle By Name(w596) -> ("root"=w594:T2, "Error Log"=w595:refnum<file>, "standard events"=w590:T3)
        n243 = call "ClearStandardEvents.vi"("error in"=w585, "standard events"=w590, "sub panel ref in"=w592) -> ("error out"=w588:errorcluster)  [unwired: 8 in]
        n244 = Close File(refnum=w595, error in=w588) -> (error out=w589:errorcluster)  [unwired: 1 out]
        n245 = call "CloseNode.vi"("error in"=w589, "node ref"=w594) -> ("error out"=w583:errorcluster)  [unwired: 9 in]
        n246 = disable-structure shown="RUN_TIME_ENGINE==True" {
          disable-tunnel: w583 -> [w597 w598]
          disable-tunnel: [w597 w598] -> w582
          disable-tunnel: w581 -> [_ _]
          frame condition #0 (active) {
          }
          frame condition #1 {
            n247 = Quit LabVIEW() -> ()  [unwired: 1 in]
          }
        }
      }
      frame "------------Menu Operations--------------" {
        # "Dummy case to add a seperation in the Case Structure menu"
      }
      frame "Close?", "New?", "Open?" {
        n248 = Unbundle By Name(w603) -> ("current path"=w602:path, "unsaved changes"=w604:bool, "repository"=w606:refnum<class "CEF_Repository.lvclass">, "root"=w605:T2)
        n249 = case shown="True" w604 {
          tunnel: w612 -> [w623 w631]
          tunnel: [w623 w624] -> w613
          tunnel: [TRUE ("Cancelled") w626] -> w611
          tunnel: w606 -> [_ w628]
          tunnel: w605 -> [_ w629]
          tunnel: w602 -> [_ w625]
          frame False {
            # "If there is nothing to save Go do Action"
          }
          frame True {
            n250 = call-dynamic "ReadTree.vi"("error in"=w631, "root"=w629, "CEF_Repository in"=w628) -> ("error out"=w630:errorcluster, "CEF_Repository out"=w627:refnum<class "CEF_Repository.lvclass">)  [unwired: 7 in]
            n251 = call "SaveDialog.vi"("error in"=w630, "current path"=w625, "repository"=w627) -> ("error out"=w624:errorcluster, "Done?"=w626:bool)  [unwired: 6 in, 1 out]
          }
        }
        n252 = Search and Replace String(input string=w610, search string="?", replace string="") -> (result string=w601:string)  [unwired: 5 in, 3 out]
        n253 = case shown="True" w611 {
          tunnel: [w615 w620] -> w614
          tunnel: w613 -> [w615 w621]
          tunnel: w607 -> [_ w619]
          tunnel: w601 -> [_ w618]
          frame False {
          }
          frame True {
            n254 = Bundle("result string"=w618, "") -> (w616:cluster{"result string":string, string})  [unwired: 1 in]
            n255 = Enqueue Element(queue=w619, element=w616, error in (no error)=w621) -> (error out=w620:errorcluster)  [unwired: 1 in, 2 out]
          }
        }
      }
      frame "New" {
        n256 = case shown="False" w635 {
          tunnel: w644 -> [w661 _]
          tunnel: w643 -> [w657 w665]
          tunnel: w642 -> [w655 w668]
          tunnel: [w649 w667] -> w640
          tunnel: [w651 path "" ("Configuration file")] -> w636
          tunnel: w647 -> [w658 _]
          tunnel: w634 -> [_ _]
          frame False {
            n257 = Unbundle By Name(w658) -> ("paths.Configuration"=w651:path)
            n258 = Bundle("notification"="Open", "") -> (w656:cluster{"notification":string, string})  [unwired: 1 in]
            n259 = Enqueue Element(queue=w657, element=w656, error in (no error)=w655) -> (error out=w652:errorcluster)  [unwired: 1 in, 2 out]
            n260 = Path To String(path=w651) -> (string=w650:string)
            n261 = Bundle("notification"="Open Config", w650) -> (w659:cluster{"notification":string, string})  [unwired: 1 in]
            n262 = Send Notification(notification=w659, notifier=w661, error in (no error)=w652) -> (error out=w649:errorcluster)  [unwired: 1 out]
          }
          frame True {
            n263 = Bundle("PopulateTree", "") -> (w662:cluster{string, string})  [unwired: 1 in]
            n264 = Enqueue Element(queue=w665, element=w662, error in (no error)=w668) -> (error out=w667:errorcluster)  [unwired: 1 in, 2 out]
          }
        }
        n265 = Unbundle By Name(w647) -> ("paths.Plugin"=w641:path)
        n266 = call-dynamic "Initialize.vi"("error in"=w640, "path"=w641, "CEF_Repository in"=refnum<class "CEF_HierarchyRepo.lvclass"> refnum ("CEF.lvlibp:CEF_HierarchyRepo.lvclass")) -> ("error out"=w645:errorcluster, "CEF_Repository out"=w637:refnum<class "CEF_HierarchyRepo.lvclass">)  [unwired: 7 in]
        n267 = call-dynamic "Initialize.vi"("error in"=w645, "CEF_Serialize node in"=refnum<class "System.lvclass"> refnum ("System.lvlibp:System")) -> ("error out"=w632:errorcluster, "data value reference"=w639:refnum<data-value>)  [unwired: 7 in, 1 out]
        n268 = Bundle By Name(cluster=w647, "unsaved changes"=FALSE, "current path"=w636, "repository"=w637, "root"=w639) -> (w648:T1)
      }
      frame "Open" {
        n269 = Unbundle By Name(w691) -> ("unsaved changes"=w686:bool, "root"=w685:T2, "repository"=w676:refnum<class "CEF_Repository.lvclass">, "current path"=w677:path, "paths.Configuration"=w680:path)
        n270 = case shown="True" w671 {
          tunnel: w670 -> [w692 w694]
          tunnel: [w692 w693] -> w669
          frame False {
          }
          frame True {
            n271 = invoke class="VI" method="FP.Open"(error in=w694) -> (error out=w693:errorcluster)  [unwired: 4 in, 4 out]
          }
        }
        n272 = Equal?(x=w680, y=path "" ("f")) -> (x = y?=w681:bool)
        n273 = Not(x=w681) -> (.not. x?=w683:bool)
        n274 = Not(x=w671) -> (.not. x?=w672:bool)
        n275 = And(x=w683, y=w672) -> (x .and. y?=w674:bool)
        n276 = case shown="False" w674 {
          tunnel: [w697 w698] -> w689
          tunnel: [w696 _] -> w688
          tunnel: w680 -> [w695 w698]
          frame False {
            n277 = call "FileDialog.vi"("start path"=w695) -> ("cancelled"=w696:bool, "selected path"=w697:path)  [unwired: 8 in, 1 out]
          }
          frame True {
          }
        }
        n278 = case shown="False" w688 {
          tunnel: [w700 w733] -> w675
          tunnel: w669 -> [w713 w733]
          tunnel: w685 -> [w708 w734]
          tunnel: [w706 w735] -> w679
          tunnel: w689 -> [w709 w735]
          tunnel: w686 -> [_ w736]
          tunnel: [FALSE ("unsaved changes") w736] -> w687
          tunnel: [w707 w734] -> w684
          tunnel: w677 -> [w705 _]
          tunnel: w676 -> [w703 w732]
          tunnel: [w704 w732] -> w678
          tunnel: w672 -> [w702 _]
          tunnel: w673 -> [w701 _]
          frame False {
            n279 = call-dynamic "Open.vi"("error in"=w713, "file path"=w709, "CEF_Repository in"=w703) -> ("error out"=w711:errorcluster, "invalid?"=w712:bool, "CEF_Repository out"=w710:refnum<class "CEF_Repository.lvclass">)  [unwired: 6 in]
            n280 = case shown="False" w712 {
              tunnel: [w724 w731] -> w704
              tunnel: [w715 w727] -> w700
              tunnel: [w721 w730] -> w707
              tunnel: w710 -> [w723 w731]
              tunnel: w711 -> [w720 w727]
              tunnel: w709 -> [w722 _]
              tunnel: w708 -> [_ w730]
              tunnel: [w722 w729] -> w706
              tunnel: w705 -> [_ w729]
              tunnel: w702 -> [w718 _]
              tunnel: [w716 w725] -> w699
              frame False {
                n281 = call-dynamic "WriteTree.vi"("error in"=w720, "CEF_Repository in"=w723) -> ("error out"=w715:errorcluster, "root"=w721:refnum<data-value>, "CEF_Repository out"=w724:refnum<class "CEF_Repository.lvclass">)  [unwired: 7 in]
                n282 = Flatten To String(anything=w718) -> (data string=w717:string)  [unwired: 3 in, 2 out]
                n283 = Bundle("Control Engines", "data string"=w717) -> (w716:cluster{string, "data string":string})  [unwired: 1 in]
              }
              frame True {
                n284 = Bundle("notification"="PopulateTree", "") -> (w725:cluster{"notification":string, string})  [unwired: 1 in]
              }
            }
            n285 = Enqueue Element(queue=w701, element=w699) -> ()  [unwired: 2 in, 3 out]
          }
          frame True {
          }
        }
        n286 = Bundle By Name(cluster=w691, "unsaved changes"=w687, "root"=w684, "repository"=w678, "current path"=w679, "paths.Configuration"=w679) -> (w690:T1)
      }
      frame "Save" {
        n287 = Unbundle By Name(w746) -> ("current path"=w747:path, "repository"=w737:refnum<class "CEF_Repository.lvclass">, "root"=w748:T2)
        n288 = Empty String/Path?(string/path=w747) -> (empty?=w749:bool)
        n289 = Not A Number/Path/Refnum?(number/path/refnum=w747) -> (NaN/Path/Refnum?=w750:bool)
        n290 = call-dynamic "ReadTree.vi"("error in"=w738, "root"=w748, "CEF_Repository in"=w737) -> ("error out"=w744:errorcluster, "CEF_Repository out"=w743:refnum<class "CEF_Repository.lvclass">)  [unwired: 7 in]
        n291 = Or(x=w749, y=w750) -> (x .or. y?=w751:bool)
        n292 = case shown="True" w751 {
          tunnel: w747 -> [w754 w764]
          tunnel: [w754 w763] -> w739
          tunnel: w744 -> [w756 w758]
          tunnel: w743 -> [w755 w761]
          tunnel: [w752 w760] -> w742
          tunnel: [w753 w759] -> w741
          frame False {
            # "unchanged file path"
            n293 = call-dynamic "Save.vi"("error in"=w756, "file path"=w754, "CEF_Repository in"=w755) -> ("error out"=w753:errorcluster, "CEF_Repository out"=w752:refnum<class "CEF_Repository.lvclass">)  [unwired: 7 in]
          }
          frame True {
            # "Empthy path, Not a Path, and changed"
            n294 = call "FileDialog.vi"("error in"=w758, "start path"=w764) -> ("error out"=w757:errorcluster, "cancelled"=w765:bool, "selected path"=w762:path)  [unwired: 7 in]
            n295 = case shown="False" w765 {
              tunnel: [w768 w773] -> w763
              tunnel: w762 -> [w768 w773]
              tunnel: w757 -> [w770 w771]
              tunnel: w761 -> [w769 w772]
              tunnel: [w767 w772] -> w760
              tunnel: [w766 w771] -> w759
              frame False {
                n296 = call-dynamic "Save.vi"("error in"=w770, "file path"=w768, "CEF_Repository in"=w769) -> ("error out"=w766:errorcluster, "CEF_Repository out"=w767:refnum<class "CEF_Repository.lvclass">)  [unwired: 7 in]
              }
              frame True {
              }
            }
          }
        }
        n297 = Unbundle By Name(w741) -> ("status"=w740:bool)
        n298 = Bundle By Name(cluster=w746, "paths.Configuration"=w739, "current path"=w739, "repository"=w742, "unsaved changes"=w740) -> (w745:T1)
      }
      frame "SaveAs" {
        n299 = Unbundle By Name(w780) -> ("current path"=w781:path, "repository"=w775:refnum<class "CEF_Repository.lvclass">, "root"=w786:T2)
        n300 = call-dynamic "ReadTree.vi"("error in"=w776, "root"=w786, "CEF_Repository in"=w775) -> ("error out"=w783:errorcluster, "CEF_Repository out"=w782:refnum<class "CEF_Repository.lvclass">)  [unwired: 7 in]
        n301 = call "FileDialog.vi"("error in"=w783, "start path"=w781) -> ("error out"=w784:errorcluster, "cancelled"=w785:bool, "selected path"=w774:path)  [unwired: 7 in]
        n302 = case shown="False" w785 {
          tunnel: w774 -> [w789 _]
          tunnel: w784 -> [w791 w792]
          tunnel: w782 -> [w790 w793]
          tunnel: [w788 w793] -> w779
          tunnel: [w787 w792] -> w778
          frame False {
            n303 = call-dynamic "Save.vi"("error in"=w791, "file path"=w789, "CEF_Repository in"=w790) -> ("error out"=w787:errorcluster, "CEF_Repository out"=w788:refnum<class "CEF_Repository.lvclass">)  [unwired: 7 in]
          }
          frame True {
          }
        }
        n304 = Bundle By Name(cluster=w780, "paths.Configuration"=w774, "current path"=w774, "repository"=w779) -> (w777:T1)
      }
      frame "-------TreeControl Operations-----------" {
        # "Dummy case to add a seperation in the Case Structure menu"
      }
      frame "AddNode" {
        n305 = Unbundle By Name(w824) -> ("glyph manager"=w823:T5, "repository"=w810:refnum<class "CEF_Repository.lvclass">)
        n306 = Unflatten From String(type=T8 {"subNode"="", "Node ID"=""} ("input cluster"), binary string=w816, error in (no error)=w817) -> (value=w818:T8, error out=w812:errorcluster)  [unwired: 2 in, 1 out]
        n307 = Unbundle By Name(w818) -> ("Node ID"=w815:string, "subNode"=w806:string)
        n308 = call-dynamic "GetClassPath.vi"("error in"=w812, "class name"=w806, "CEF_Repository in"=w810) -> ("error out"=w808:errorcluster, "class path"=w811:path)  [unwired: 6 in, 1 out]
        n309 = call <vilib>:"Get LV Class Default Value.vi"("error in (no error)"=w808, "class path"=w811) -> ("error out"=w807:errorcluster, "object"=w809:refnum<class>)  [unwired: 8 in]
        n310 = To More Specific Class(target class=refnum<class "CEF_serializable node.lvclass"> refnum ("CEF.lvlibp:CEF_serializable node.lvclass"), reference=w809, error in=w807) -> (specific class reference=w813:refnum<class "CEF_serializable node.lvclass">, error out=w814:errorcluster)
        n311 = call "AddNode.vi"("error in"=w814, "parameters"=w806, "parent node ID"=w815, "CEF_Node in"=w813) -> ("error out"=w822:errorcluster, "summary"=w804:T18)  [unwired: 6 in]
        n312 = call "PopulateTreeSumaryWithGlyphManager.vi"("error in"=w822, "glyph manager"=w823, "summary"=w804, "tree ref in"=w796) -> ("error out"=w803:errorcluster, "glyph manager out"=w820:T17)  [unwired: 6 in]
        n313 = Index Array(array=w804) -> (element=w805:T19)  [unwired: 1 in]
        n314 = Unbundle By Name(w805) -> ("ID"=w799:string)
        n315 = Bundle By Name(cluster=w824, "unsaved changes"=TRUE, "glyph manager"=w820) -> (w825:T1)
        n316 = Bundle("format string"="RefreshNode", "ID"=w799) -> (w797:cluster{"format string":string, "ID":string})  [unwired: 1 in]
        n317 = Enqueue Element(queue=w798, element=w797, error in (no error)=w803) -> (error out=w802:errorcluster)  [unwired: 1 in, 2 out]
      }
      frame "Duplicate" {
        n318 = Unbundle By Name(w833) -> ("glyph manager"=w830:T5)
        n319 = call "IDtoNode.vi"("error in"=w827, "ID"=w828) -> ("error out"=w835:errorcluster, "invalid Id"=w834:bool, "node ref"=w836:refnum<data-value>)  [unwired: 7 in]
        n320 = case shown="False" w834 {
          tunnel: [w848 w850] -> w837
          tunnel: w836 -> [w847 _]
          tunnel: w835 -> [w844 w851]
          tunnel: w830 -> [w840 w854]
          tunnel: [w839 w854] -> w829
          tunnel: w826 -> [w838 _]
          frame False {
            n321 = call "DuplicateNode.vi"("same parent?"=TRUE ("s"), "error in"=w844, "node ref in"=w847) -> ("error out"=w845:errorcluster, "new node ref"=w846:refnum<data-value>)  [unwired: 7 in]
            n322 = call "Summary.vi"("error in"=w845, "node self ref"=w846) -> ("error out"=w842:errorcluster, "summary"=w841:T18)  [unwired: 8 in]
            n323 = call "PopulateTreeSumaryWithGlyphManager.vi"("error in"=w842, "glyph manager"=w840, "summary"=w841, "tree ref in"=w838) -> ("error out"=w848:errorcluster, "glyph manager out"=w839:T17)  [unwired: 6 in]
          }
          frame True {
            n324 = call "CEF_error generator.vi"("error in"=w851, "source"="TSS::Duplicate", "append error message"="Node invalid " ("source"), "error code (0)"=42) -> ("error out"=w850:errorcluster)  [unwired: 5 in]
          }
        }
        n325 = Bundle By Name(cluster=w833, "unsaved changes"=TRUE, "glyph manager"=w829) -> (w832:T1)
      }
      frame "CustomMenuAction" {
        n326 = Unbundle By Name(w862) -> ("standard events.node change"=w859:refnum<user-event>)
        n327 = Match Pattern(string=w863, regular expression=":") -> (before substring=w866:string, after substring=w860:string)  [unwired: 1 in, 2 out]
        n328 = call "IDtoNode.vi"("error in"=w857, "ID"=w860) -> ("error out"=w856:errorcluster, "invalid Id"=w867:bool, "node ref"=w868:refnum<data-value>)  [unwired: 7 in]
        n329 = case shown="False" w867 {
          tunnel: [w880 w914] -> w864
          tunnel: w868 -> [w878 _]
          tunnel: w856 -> [w874 w915]
          tunnel: w866 -> [w881 _]
          tunnel: w858 -> [w879 _]
          tunnel: w861 -> [w876 _]
          tunnel: w859 -> [w872 _]
          tunnel: w855 -> [w869 _]
          frame False {
            n330 = in-place {
              in-place-border: [w911] -> w882
              in-place-border: w881 -> [w907]
              in-place-border: w879 -> [w910]
              in-place-border: [w909] -> w877
              in-place-border: w876 -> [w903]
              in-place-border: [w907] -> w875
              in-place-border: w874 -> [w906]
              in-place-border: [w905] -> w873
              in-place-border: w872 -> [w904]
              in-place-border: [w904] -> w871
              in-place-border: w869 -> [w902]
              n331 = in-place-dvr #5(w878) -> (w908:refnum<class "CEF_Node.lvclass">)  [unwired: 1 out]
              n332 = call-dynamic "MenuHandler.vi"("tree control"=w910, "main queue"=w903, "error in"=w906, "parameters"=w902, "menu string"=w907, "CEF_Node in"=w908) -> ("error out"=w905:errorcluster, "refresh tree?"=w909:bool, "Unhandled"=w911:bool, "CEF_Node out"=w912:refnum<class "CEF_Node.lvclass">)  [unwired: 2 in]
              n333 = in-place-dvr #5(w912) -> (w870:refnum<data-value>)  [unwired: 1 out]
            }
            n334 = case shown="False" w882 {
              tunnel: w875 -> [_ w893]
              tunnel: [w887 w894] -> w880
              tunnel: w873 -> [w885 w895]
              tunnel: w877 -> [w886 _]
              tunnel: w871 -> [w884 _]
              tunnel: w870 -> [w883 _]
              frame False {
                n335 = case shown="True" w886 {
                  tunnel: [w888 w889] -> w887
                  tunnel: w885 -> [w888 w890]
                  tunnel: w884 -> [_ w892]
                  tunnel: w883 -> [_ w891]
                  frame False {
                  }
                  frame True {
                    # "update EngineMap"
                    n336 = Generate User Event(user event=w892, event data cluster=w891, error in=w890) -> (error out=w889:errorcluster)  [unwired: 1 in, 1 out]
                  }
                }
              }
              frame True {
                n337 = disable-structure shown="Default" {
                  disable-tunnel: w895 -> [w898 w901]
                  disable-tunnel: [w897 w901] -> w894
                  disable-tunnel: w893 -> [w896 _]
                  frame condition #0 {
                    n338 = call "CEF_error generator.vi"("error in"=w898, "source"="TSS::CustomMenuAction", "append error message"=w896, "error code (0)"=538506) -> ("error out"=w897:errorcluster)  [unwired: 5 in]
                  }
                  frame condition #1 (active) {
                  }
                }
              }
            }
          }
          frame True {
            n339 = call "CEF_error generator.vi"("error in"=w915, "source"="TSS:CustomMenuAction", "append error message"="Node invalid " ("source"), "error code (0)"=42) -> ("error out"=w914:errorcluster)  [unwired: 5 in]
          }
        }
      }
      frame "RefreshNode" {
        # "Refreshes the node in the Tree, Sets the save flag to true. This case can be called from the UIs of the nodes"
        n340 = Unbundle By Name(w932) -> ("glyph manager"=w923:T5, "root"=w919:T2)
        n341 = call "IDtoNode.vi"("error in"=w934, "ID"=w925) -> ("error out"=w924:errorcluster, "invalid Id"=w928:bool, "node ref"=w927:refnum<data-value>)  [unwired: 7 in]
        n342 = Select(t=w919, s=w928, f=w927) -> (s? t:f=w926:T2)
        n343 = call "SummaryWithGlyphManager.vi"("error in"=w924, "glyph manager"=w923, "node self ref"=w926) -> ("error out"=w922:errorcluster, "glyph manager out"=w929:T17, "summary"=w921:T18)  [unwired: 6 in]
        n344 = call "RefreshSubTreeWithGlyphManager.vi"("error in"=w922, "glyph manager"=w929, "node information"=w921, "tree ref in"=w918) -> ("error out"=w931:errorcluster, "glyph manager out"=w933:T17, "tree ref out"=w930:refnum<vi>)  [unwired: 5 in]
        n345 = Close Reference(reference=w930, error in (no error)=w931) -> (error out=w920:errorcluster)
        n346 = Bundle By Name(cluster=w932, "glyph manager"=w933) -> (w935:T1)
      }
      frame "RemoveNode" {
        n347 = call "IDtoNode.vi"("error in"=w945, "ID"=w941) -> ("error out"=w944:errorcluster, "invalid Id"=w942:bool, "node ref"=w943:refnum<data-value>)  [unwired: 7 in]
        n348 = case shown="False" w942 {
          tunnel: w944 -> [w947 w954]
          tunnel: w943 -> [w948 _]
          tunnel: [w949 w953] -> w938
          tunnel: w936 -> [w946 _]
          frame False {
            n349 = call "RemoveNode.vi"("error in"=w947, "node"=w948) -> ("error out"=w950:errorcluster, "node ID"=w951:string)  [unwired: 8 in]
            n350 = call "ClearTreeNode.vi"("error in"=w950, "tag"=w951, "tree reference"=w946) -> ("error out"=w949:errorcluster)  [unwired: 8 in]
          }
          frame True {
            n351 = call "CEF_error generator.vi"("error in"=w954, "source"="TSS:RemoveNode", "append error message"="Node invalid " ("source"), "error code (0)"=42) -> ("error out"=w953:errorcluster)  [unwired: 5 in]
          }
        }
        n352 = Bundle By Name(cluster=w937, "unsaved changes"=TRUE) -> (w939:T1)
      }
      frame "PopulateTree" {
        # "Close the Launch Panel, and show the main UI panel"
        n353 = call <vilib>:"Set Busy.vi"("error in (no error)"=w972) -> ("error out"=w962:errorcluster)  [unwired: 9 in, 1 out]
        n354 = case shown="False" w964 {
          tunnel: w963 -> [w984 _]
          tunnel: w962 -> [w981 w985]
          tunnel: [w980 w985] -> w961
          frame False {
            n355 = Bundle("notification"="Launched", "") -> (w982:cluster{"notification":string, string})  [unwired: 1 in]
            n356 = Send Notification(notification=w982, notifier=w984, error in (no error)=w981) -> (error out=w980:errorcluster)  [unwired: 1 out]
          }
          frame True {
          }
        }
        n357 = Unbundle By Name(w978) -> ("root"=w969:T2, "glyph manager"=w966:T5, "standard events.user event"=w973:refnum<user-event>)
        n358 = call "ClearSubPanel.vi"("error in"=w961, "user event ref"=w973, "sub panel ref in"=w967) -> ("error out"=w970:errorcluster)  [unwired: 7 in, 1 out]
        n359 = call "SummaryWithGlyphManager.vi"("error in"=w970, "glyph manager"=w966, "node self ref"=w969) -> ("error out"=w957:errorcluster, "glyph manager out"=w971:T17, "summary"=w958:T18)  [unwired: 6 in]
        n360 = case shown="\"\"" w975 {
          selector: w975 -> [w986 _]
          tunnel: w958 -> [_ w988]
          tunnel: [w986 w987] -> w974
          frame Default {
          }
          frame "" {
            n361 = Index Array(array=w988) -> (element=w989:T19)  [unwired: 1 in]
            n362 = Unbundle By Name(w989) -> ("ID"=w987:string)
          }
        }
        n363 = property class="Tree (strict)"(reference=w968, "Val(Sgnl)"=w974) -> (reference out=w960:refnum<vi>)  [unwired: 1 in, 1 out]
        n364 = call "RefreshEntireTreeWithGlyphManager.vi"("calling VI"=w965, "error in"=w957, "glyph manager"=w971, "array"=w958, "tree ref in"=w960) -> ("error out"=w959:errorcluster, "glyph manager out"=w976:T17)  [unwired: 5 in]
        n365 = Bundle By Name(cluster=w978, "glyph manager"=w976) -> (w977:T1)
      }
      frame "ActivateNode" {
        n366 = Unbundle By Name(w1001) -> ("standard events"=w995:T3)
        n367 = property class="Pnl"(reference=w990, "DeferPanUpdts"=TRUE ("Defer Panel Updates")) -> (reference out=w993:refnum<vi>)  [unwired: 1 in, 1 out]
        n368 = call "IDtoNode.vi"("error in"=w992, "ID"=w994) -> ("error out"=w999:errorcluster, "invalid Id"=w1002:bool, "node ref"=w1000:refnum<data-value>)  [unwired: 7 in]
        n369 = case shown="False" w1002 {
          tunnel: w1000 -> [w1013 _]
          tunnel: [w1007 w1018] -> w997
          tunnel: w999 -> [w1005 w1019]
          tunnel: w995 -> [w1003 _]
          tunnel: w991 -> [w1011 _]
          tunnel: w998 -> [w1009 _]
          tunnel: w993 -> [w1012 _]
          tunnel: w994 -> [_ w1016]
          frame False {
            n370 = Unbundle By Name(w1003) -> ("user event"=w1010:refnum<user-event>)
            n371 = call "ClearSubPanel.vi"("error in"=w1005, "user event ref"=w1010, "sub panel ref in"=w1011) -> ("error out"=w1004:errorcluster)  [unwired: 7 in, 1 out]
            n372 = call "LoadNodeUIStandardEvents.vi"("Standard Event"=w1003, "error in"=w1004, "sub panel ref"=w1011, "main queue"=w1009, "node"=w1013) -> ("error out"=w1008:errorcluster)  [unwired: 6 in]
            n373 = property class="Pnl"(reference=w1012, error in=w1008, "DeferPanUpdts"=FALSE ("Defer Panel Updates")) -> (error out=w1007:errorcluster)  [unwired: 1 out]
          }
          frame True {
            n374 = Format Into String(format string="%s node is invalid" ("initial string"), w1016) -> (resulting string=w1014:string)  [unwired: 2 in, 1 out]
            n375 = call "CEF_error generator.vi"("error in"=w1019, "source"="TSS::ActivateNode", "append error message"=w1014, "error code (0)"=42) -> ("error out"=w1018:errorcluster)  [unwired: 5 in]
          }
        }
      }
      frame "Move" {
        n376 = Unflatten From String(type=T9 {"node ref"=refnum, "new parent"=refnum, "Index"=0} ("Cluster"), binary string=w1039, error in (no error)=w1036) -> (value=w1037:T9, error out=w1032:errorcluster)  [unwired: 2 in, 1 out]
        n377 = Unbundle By Name(w1037) -> ("Index"=w1021:i32, "node ref"=w1028:T2, "new parent"=w1040:T2)
        n378 = call "MoveNode.vi"("error in"=w1032, "index"=w1021, "new parent"=w1040, "node"=w1028) -> ("error out"=w1030:errorcluster)  [unwired: 7 in]
        n379 = call "Summary.vi"("error in"=w1030, "node self ref"=w1028) -> ("error out"=w1029:errorcluster, "summary"=w1026:T18)  [unwired: 8 in]
        n380 = Index Array(array=w1026, index=w1021) -> (element=w1027:T19)
        n381 = Unbundle By Name(w1027) -> ("ID"=w1024:string)
        n382 = Bundle By Name(cluster=w1033, "unsaved changes"=TRUE) -> (w1034:T1)
        n383 = Bundle("PopulateTree", "ID"=w1024) -> (w1022:cluster{string, "ID":string})  [unwired: 1 in]
        n384 = Enqueue Element(queue=w1023, element=w1022, error in (no error)=w1029) -> (error out=w1031:errorcluster)  [unwired: 1 in, 2 out]
      }
      frame "NodeDataChange" {
        n385 = Unbundle By Name(w1056) -> ("root"=w1043:T2)
        n386 = property class="NISE_CEF_Node"(reference=w1043) -> ("DataAccess:Children"=w1044:refnum<data-value>[])  [unwired: 1 in, 2 out]
        n387 = Index Array(array=w1044) -> (element=w1042:refnum<data-value>)  [unwired: 1 in]
        n388 = call "Find Engine from Child.vi"("error in (no error)"=w1054, "Node ID"=w1055, "HW Engine"=w1042) -> ("error out"=w1048:errorcluster, "Engine"=w1053:refnum<data-value>)  [unwired: 7 in]
        n389 = in-place {
          in-place-border: w1045 -> [w1065]
          in-place-border: w1049 -> [w1062]
          in-place-border: w1048 -> [w1064]
          in-place-border: [w1063] -> w1047
          in-place-border: [w1062] -> w1046
          in-place-border: w1041 -> [w1060]
          n390 = in-place-dvr #6(w1053) -> (w1066:refnum<class "CEF_Node.lvclass">)  [unwired: 1 out]
          n391 = call-dynamic "MenuHandler.vi"("tree control"=w1065, "main queue"=w1062, "error in"=w1064, "parameters"=w1060, "menu string"="Reset Engine" ("message value"), "CEF_Node in"=w1066) -> ("error out"=w1063:errorcluster, "CEF_Node out"=w1067:refnum<class "CEF_Node.lvclass">)  [unwired: 2 in, 2 out]
          n392 = in-place-dvr #6(w1067) -> ()  [unwired: 2 out]
        }
        n393 = Bundle By Name(cluster=w1056, "unsaved changes"=TRUE) -> (w1059:T1)
        n394 = Bundle("message name"="RefreshNode", "") -> (w1050:cluster{"message name":string, string})  [unwired: 1 in]
        n395 = Enqueue Element(queue=w1046, element=w1050, error in (no error)=w1047) -> (error out=w1057:errorcluster)  [unwired: 1 in, 2 out]
      }
      frame "-------Engine Operations-----------" {
      }
      frame "Export Engine" {
        n396 = Unbundle By Name(w1073) -> ("repository"=w1075:refnum<class "CEF_Repository.lvclass">, "current path"=w1070:path)
        n397 = call "IDtoNode.vi"("error in"=w1080, "ID"=w1079) -> ("error out"=w1076:errorcluster, "invalid Id"=w1078:bool, "node ref"=w1077:refnum<data-value>)  [unwired: 7 in]
        n398 = case shown="False" w1078 {
          tunnel: w1077 -> [w1085 _]
          tunnel: w1076 -> [w1082 w1107]
          tunnel: w1075 -> [w1090 w1104]
          tunnel: [w1088 w1106] -> w1074
          tunnel: [w1087 w1104] -> w1071
          tunnel: w1070 -> [w1086 _]
          frame False {
            n399 = property class="NISE_CEF_Node"(reference=w1085, error in=w1082) -> (reference out=w1083:refnum<data-value>, error out=w1081:errorcluster, "DataAccess:NodeClass"=w1084:string)
            n400 = call "FileDialog.vi"("error in"=w1081, "default name"=w1084, "start path"=w1086) -> ("error out"=w1091:errorcluster, "cancelled"=w1092:bool, "selected path"=w1089:path)  [unwired: 6 in]
            n401 = case shown="False" w1092 {
              tunnel: w1091 -> [w1100 w1101]
              tunnel: w1083 -> [w1099 _]
              tunnel: w1090 -> [w1098 w1102]
              tunnel: w1089 -> [w1093 _]
              tunnel: [w1095 w1101] -> w1088
              tunnel: [w1094 w1102] -> w1087
              frame False {
                n402 = call-dynamic "ReadTree.vi"("error in"=w1100, "root"=w1099, "CEF_Repository in"=w1098) -> ("error out"=w1096:errorcluster, "CEF_Repository out"=w1097:refnum<class "CEF_Repository.lvclass">)  [unwired: 7 in]
                n403 = call-dynamic "Save.vi"("error in"=w1096, "file path"=w1093, "CEF_Repository in"=w1097) -> ("error out"=w1095:errorcluster, "CEF_Repository out"=w1094:refnum<class "CEF_Repository.lvclass">)  [unwired: 7 in]
              }
              frame True {
              }
            }
          }
          frame True {
            n404 = call "CEF_error generator.vi"("error in"=w1107, "source"="TSS::Export Engine", "append error message"="Invalid Node" ("source"), "error code (0)"=42) -> ("error out"=w1106:errorcluster)  [unwired: 5 in]
          }
        }
        n405 = Bundle By Name(cluster=w1073, "repository"=w1071) -> (w1072:T1)
      }
      frame "Import Engine" {
        n406 = Unbundle By Name(w1120) -> ("root"=w1111:T2, "repository"=w1123:refnum<class "CEF_Repository.lvclass">, "current path"=w1116:path)
        n407 = call "IDtoNode.vi"("error in"=w1115, "ID"=w1110) -> ("error out"=w1114:errorcluster, "node ref"=w1113:refnum<data-value>)  [unwired: 7 in, 1 out]
        n408 = call "FileDialog.vi"("error in"=w1114, "start path"=w1116) -> ("error out"=w1124:errorcluster, "cancelled"=w1117:bool, "selected path"=w1121:path)  [unwired: 7 in]
        n409 = case shown="True" w1117 {
          tunnel: w1124 -> [w1135 w1167]
          tunnel: w1123 -> [w1134 w1166]
          tunnel: w1122 -> [w1131 _]
          tunnel: w1121 -> [w1127 _]
          tunnel: [w1130 w1165] -> w1112
          tunnel: [w1129 w1166] -> w1109
          tunnel: [w1128 w1167] -> w1118
          tunnel: w1113 -> [w1126 _]
          tunnel: w1111 -> [w1125 w1165]
          frame False {
            n410 = call-dynamic "Open.vi"("error in"=w1135, "file path"=w1127, "CEF_Repository in"=w1134) -> ("error out"=w1132:errorcluster, "invalid?"=w1136:bool, "CEF_Repository out"=w1133:refnum<class "CEF_Repository.lvclass">)  [unwired: 6 in]
            n411 = case shown="False" w1136 {
              tunnel: [w1154 w1155] -> w1129
              tunnel: [w1151 w1163] -> w1128
              tunnel: [w1142 w1158] -> w1130
              tunnel: w1133 -> [w1152 w1155]
              tunnel: w1132 -> [w1153 w1164]
              tunnel: w1131 -> [w1137 _]
              tunnel: w1127 -> [_ w1160]
              tunnel: w1126 -> [w1150 _]
              tunnel: w1125 -> [w1147 w1158]
              frame False {
                n412 = call-dynamic "WriteTree.vi"("error in"=w1153, "CEF_Repository in"=w1152) -> ("error out"=w1148:errorcluster, "root"=w1149:refnum<data-value>, "CEF_Repository out"=w1154:refnum<class "CEF_Repository.lvclass">)  [unwired: 7 in]
                n413 = call "LinkNodes.vi"("error in"=w1148, "child in"=w1149, "parent in"=w1150) -> ("error out"=w1146:errorcluster, "parent out"=w1144:refnum<data-value>)  [unwired: 6 in, 1 out]
                n414 = call "LinkNodes.vi"("error in"=w1146, "child in"=w1144, "parent in"=w1147) -> ("error out"=w1145:errorcluster, "parent out"=w1143:refnum<data-value>)  [unwired: 6 in, 1 out]
                n415 = Bundle("PopulateTree", "") -> (w1138:cluster{string, string})  [unwired: 1 in]
                n416 = call "UnlinkNode.vi"("error in"=w1145, "child in"=w1144, "parent in"=w1143) -> ("error out"=w1141:errorcluster, "parent out"=w1142:refnum<data-value>)  [unwired: 6 in, 1 out]
                n417 = Enqueue Element(queue=w1137, element=w1138, error in (no error)=w1141) -> (error out=w1151:errorcluster)  [unwired: 1 in, 2 out]
              }
              frame True {
                n418 = Strip Path(path=w1160) -> (name=w1159:string)  [unwired: 1 out]
                n419 = Format Into String(format string="%s config invalid " ("source"), w1159) -> (resulting string=w1157:string)  [unwired: 2 in, 1 out]
                n420 = call "CEF_error generator.vi"("error in"=w1164, "source"="TSS::Import Engine", "append error message"=w1157, "error code (0)"=42) -> ("error out"=w1163:errorcluster)  [unwired: 5 in]
              }
            }
          }
          frame True {
          }
        }
        n421 = Bundle By Name(cluster=w1120, "repository"=w1109, "root"=w1112) -> (w1119:T1)
      }
      frame "Control Engines" {
        # "Engines"
        # "0 : HW Engine\n1 : Special Test"
        n422 = Unbundle By Name(w1186) -> ("root"=w1187:T2)
        n423 = Unflatten From String(type=TRUE, binary string=w1179, error in (no error)=w1180) -> (value=w1177:bool, error out=w1173:errorcluster)  [unwired: 2 in, 1 out]
        n424 = property class="NISE_CEF_Node"(reference=w1187) -> ("DataAccess:Children"=w1185:refnum<data-value>[])  [unwired: 1 in, 2 out]
        n425 = Index Array(array=w1185) -> (element=w1184:refnum<data-value>)  [unwired: 1 in]
        n426 = Bundle("PopulateTree", "") -> (w1176:cluster{string, string})  [unwired: 1 in]
        n427 = property class="NISE_CEF_Node"(reference=w1184) -> ("DataAccess:Children"=w1183:refnum<data-value>[])  [unwired: 1 in, 2 out]
        n428 = Enqueue Element(queue=w1171, element=w1176, error in (no error)=w1173) -> (error out=w1172:errorcluster)  [unwired: 1 in, 2 out]
        n429 = for {
          tunnel: w1183 -> [w1194] mode=indexing
          shift-right: [w1197] -> w1170
          shift-left: w1172 -> [w1193]
          tunnel: w1182 -> [w1195]
          tunnel: w1181 -> [w1192]
          tunnel: w1171 -> [w1196]
          tunnel: w1177 -> [w1191]
          n430 = in-place {
            in-place-border: w1193 -> [w1198]
            in-place-border: [w1203] -> w1197
            in-place-border: w1196 -> [w1201]
            in-place-border: w1195 -> [w1205]
            in-place-border: w1192 -> [w1202]
            in-place-border: w1191 -> [w1199]
            n431 = in-place-dvr #7(w1194) -> (w1206:refnum<class "CEF_Node.lvclass">)  [unwired: 1 out]
            n432 = case shown="True" w1199 {
              tunnel: ["Reset Engine" ("message value") "Initialize Engine" ("message value")] -> w1200
              frame False {
              }
              frame True {
                n433 = Wait (ms)(milliseconds to wait=u32 300) -> ()  [unwired: 1 out]
              }
            }
            n434 = call-dynamic "MenuHandler.vi"("tree control"=w1205, "main queue"=w1201, "error in"=w1198, "parameters"=w1202, "menu string"=w1200, "CEF_Node in"=w1206) -> ("error out"=w1203:errorcluster, "CEF_Node out"=w1204:refnum<class "CEF_Node.lvclass">)  [unwired: 2 in, 2 out]
            n435 = in-place-dvr #7(w1204) -> ()  [unwired: 2 out]
          }
        }
        n436 = case shown="False" w1169 {
          tunnel: w1170 -> [w1189 w1190]
          tunnel: [w1188 w1190] -> w1168
          frame False {
            n437 = invoke class="VI" method="FP.Open"(error in=w1189) -> (error out=w1188:errorcluster)  [unwired: 4 in, 4 out]
          }
          frame True {
          }
        }
      }
      frame "Record Engines" {
        n438 = Unflatten From String(type=TRUE, binary string=w1217, error in (no error)=w1218) -> (value=w1216:bool, error out=w1215:errorcluster)  [unwired: 2 in, 1 out]
        n439 = case shown="False" w1216 {
          selector: w1216 -> [_ w1239]
          tunnel: w1215 -> [w1226 w1231]
          tunnel: [w1222 w1237] -> w1214
          tunnel: w1213 -> [w1225 w1241]
          tunnel: [w1224 w1240] -> w1212
          tunnel: w1211 -> [_ _]
          tunnel: w1210 -> [_ _]
          frame False {
            n440 = Unbundle By Name(w1225) -> ("tdms file"=w1221:refnum<k34>)
            n441 = TDMS Close(8:w1226, 11:w1221) -> (0:w1222:errorcluster)  [unwired: 1 out]
            n442 = Bundle By Name(cluster=w1225, "tdms file"=refnum<k34> refnum, "Record"=FALSE) -> (w1224:T1)
          }
          frame True {
            n443 = Unbundle By Name(w1241) -> ("paths.Data"=w1234:path)
            n444 = Get Date/Time In Seconds() -> (seconds since 1Jan1904=w1235:timestamp)
            n445 = Format Into String(format string="%<%Y%m%d_%H%M%S>T.tdms", w1235) -> (resulting string=w1233:string)  [unwired: 2 in, 1 out]
            n446 = Build Path(base path=w1234, name or relative path=w1233) -> (appended path=w1232:path)
            n447 = TDMS Open(5:FALSE ("create index file? (T)"), 8:w1231, 10:T16."open or create" ("operation (0:open)"), 11:w1232) -> (0:w1230:errorcluster, 3:w1227:refnum<k34>)  [unwired: 3 in]
            n448 = case shown="Error .." w1230 {
              selector: w1230 -> [w1243 w1250]
              tunnel: [w1247 w1250] -> w1237
              tunnel: w1239 -> [_ w1252]
              tunnel: [TRUE ("Record") FALSE ("Record")] -> w1238
              frame No Error {
                n449 = property on="Time" class="DigNum (strict)"(error in=w1243, "Value"=0.0 ("Time")) -> (error out=w1242:errorcluster)  [unwired: 1 in, 1 out]
                n450 = call "Timing FGV.vi"("Time Target (s)"=5, "Timer Mode"=T15."Start Timer", "Error In"=w1242) -> ("Error Out"=w1247:errorcluster)  [unwired: 6 in, 2 out]
              }
              frame Error {
                n451 = Not(x=w1252) -> (.not. x?=w1251:bool)
                n452 = property on="Record" class="Bool (strict)"("Value"=w1251) -> ()  [unwired: 2 in, 2 out]
              }
            }
            n453 = Bundle By Name(cluster=w1241, "tdms file"=w1227, "Record"=w1238) -> (w1240:T1)
          }
        }
      }
    }
  }
  n454 = Merge Errors(w22, w24) -> (w23:errorcluster)
  n455 = Unregister For Events(event registration refnum=w17) -> ()  [unwired: 1 in, 1 out]
  n456 = call "DestroyStandardEvents.vi"("error in"=w23, "standard events"=w16) -> ()  [unwired: 9 in, 1 out]
